vi "4Pi Objective Lock - EMBL.vi"(7 "Calling VI Ref":refnum<vi>) -> ()   [LabVIEW 2016]
uses:
  <vilib>/Utility/miscctls.llb/LVPointTypeDef.ctl
  4Pi Objective Lock Type Defs/4Pi Obj Lock - Notifier Type.ctl
  4Pi Objective Lock Type Defs/4Pi Obj Lock - Actions.ctl
  <vilib>/vision/Image Controls.llb/IMAQ Image.ctl
  4Pi Objective Lock Type Defs/4Pi Obj Lock - Lock Settings.ctl
  Hardware Configuration/Hardware Configuration Controls/Device Type.ctl
  Hardware Configuration/Hardware Configuration Controls/Device Function.ctl
  4Pi Objective Lock Type Defs/4Pi Obj Lock - Camera Settings.ctl
  Device Library/Cameras/Camera Controls/Generic Camera ROI.ctl
  Device Library/Cameras/Camera Controls/Generic Camera Actions.ctl
  Device Library/Stages/Stages Controls/Stage Actions.ctl
  <vilib>/addons/control/pid/pid.llb/PID (DBL Array).vi
  <vilib>/addons/control/pid/pid.llb/PID (DBL).vi
  <vilib>/addons/control/pid/NI_PID_pid.lvlib
  <vilib>/vision/NI_Vision_Development_Module.lvlib
panel:
  out "dt z (s)":dbl format="%.3f"
  out "dz (µm)":dbl format="%.2f"
  out "dxy (px)":dbl[](array[numeric])
  in  "Main Tab":T1(tab)
  out "Z Move":bool
  out "XY Move":bool
  out "Measured X Position (px)":dbl=1.0 format="%.3g"
  out "Measured Y Position (px)":dbl=1.0 format="%.3g"
  out "Measured sx/sy":dbl=1.0 format="%.3g"
  out "Target X Position (px)":dbl=1.0 format="%.3g"
  out "Target Y Position (px)":dbl=1.0 format="%.3g"
  out "Target sx/sy":dbl=1.0 format="%.3g"
  out "Z Axis Position (µm)":dbl=1.0 format="%.4g"
  out "Y Axis Position (µm)":dbl=1.0 format="%.2g"
  out "X Axis Position (µm)":dbl=1.0 format="%.2g"
  out "Z Target and Fit Value (µm)":T2(graph)
  in  "Start Lock":bool
  out "Y Target and Fit Position (µm)":T2(graph)
  out "X Target and Fit Position (µm)":T2(graph)
  in  "Restart Lock":bool
  out "Fit Error":bool
  out "Move Limit Error":bool
  out "Target Z (µm)":dbl=1.0 format="%.3g"
  out "Measured Z (µm)":dbl=1.0 format="%.3g"
  out "Target X Position cc (px)":dbl=1.0 format="%.3g"
  out "Measured X Position cc (px)":dbl=1.0 format="%.3g"
  out "Measured Y Position cc (px)":dbl=1.0 format="%.3g"
  out "Target Y Position cc (px)":dbl=1.0 format="%.3g"
  in  "pixel size (µm)":dbl=0.05
  in  "X Update Scale Factor":dbl=0.01
  in  "Y Update Scale Factor":dbl=0.01
  in  "Z Update Scale Factor":dbl=0.2
  in  "Sample Z Step No.":u32=2
  in  "Sample Z Step Size (µm)":dbl=2.0
  in  "Update Delay (ms)":i32=10
  in  "D (Derivative)":dbl
  in  "I (Integral)":dbl
  in  "P (Proportional)":dbl=2.0
  in  "Invert Z Axis":bool
  in  "XY Drift Threshold":dbl=0.05
  in  "Abort If Error":bool
  in  "Flip XY Axis":bool
  in  "Invert X Axis":bool=TRUE
  in  "Invert Y Axis":bool=TRUE
  in  "Z Stage Move Limit (µm)":dbl=5.0
  in  "Z Drift Threshold":dbl=0.05
  in  "XY Stage Move Limit (µm)":dbl=1.0
  in  "Frame Accumulations":u16=10
  in  "XY Correction Active":bool=TRUE
  in  "Z Correction Active":bool=TRUE
  in  "Set Camera ROI":bool
  in  "Save Lock Settings":bool
  in  "Quit":bool
  # "Z Drift Settings"
  # "Camera Setup"
  # "XY Drift Settings"
  # "PID Control Values"
  # "General Settings"
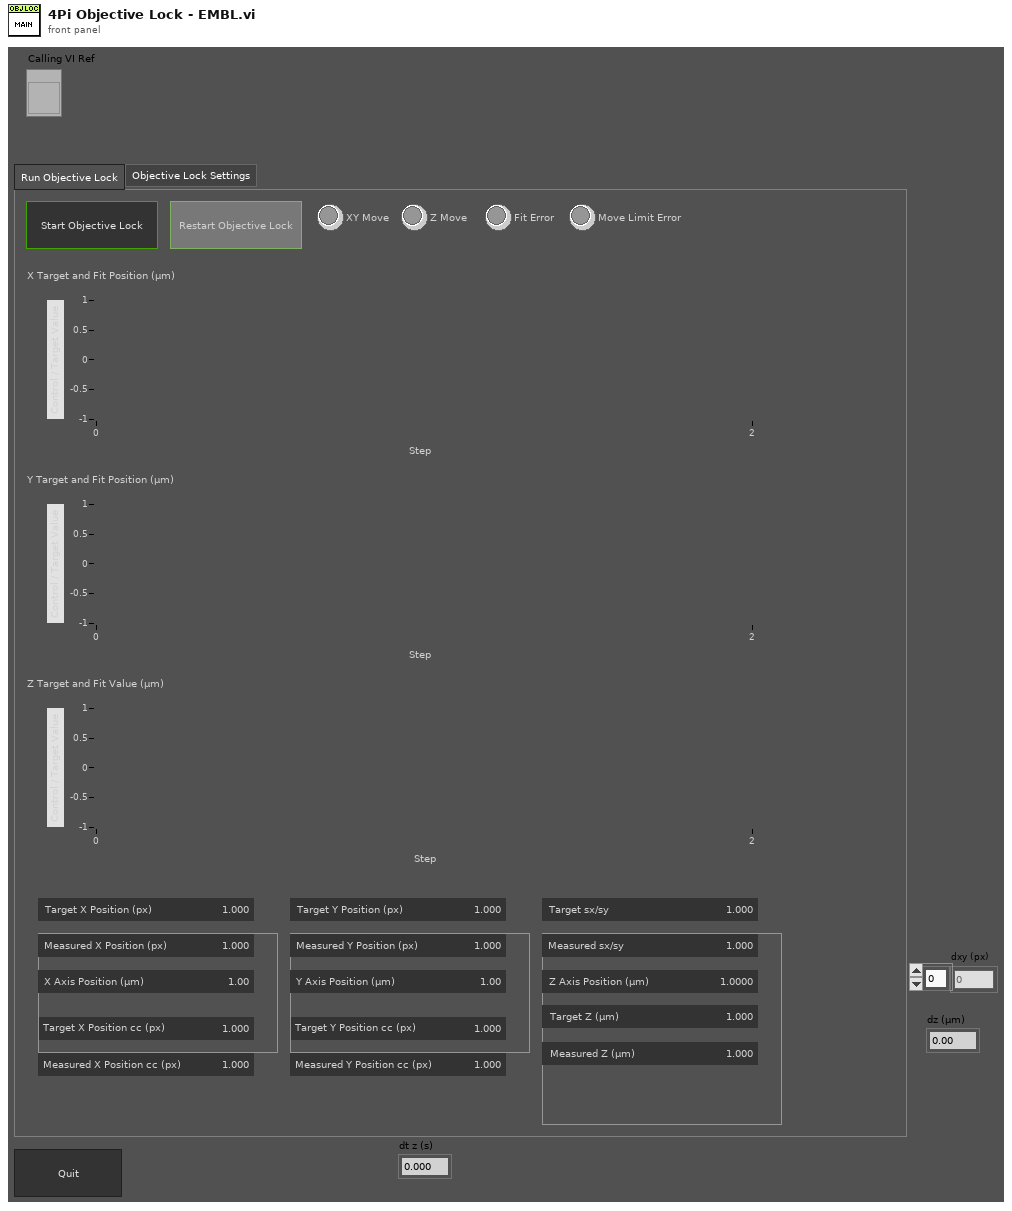
[diagram p1: front panel]
types:
  T1 = enum32{"Run Objective Lock", "Objective Lock Settings"}
  T2 = cluster{"Target 01":dbl, dbl, dbl, "Current 01":dbl, "Stage Pos":dbl, "Current 2":dbl}
  T3 = typedef "4Pi Obj Lock - Camera Settings.ctl" = cluster{"Exposure Time (s)":dbl, "H Offset":u16, "V Offset":u16, "H Width":u16, "V Width":u16}
  T4 = typedef "Device Function.ctl" = enum16{"Primary", "Secondary", "Overview", "Wide Field Drift Correction", "642 nm Excitation", "560 nm Excitation", "940 nm Excitation", "546 nm Excitation", "488 nm Excitation", "405 nm Excitation", "Objective Drift Correction", "4Pi Focus Lock", "4Pi Objective Lock", "Objective XY", "Objective Z", "Sample XY", "Sample Coarse Z", "Sample Z", "4Pi Lower", "4Pi Upper", "Em Small", "Em Large", "Ex Small", "Ex Large", "Mojo", "Adj Cavity", "Line Scanning", "Alert"}
  T5 = typedef "Device Type.ctl" = enum16{"AOTF", "Camera", "Deformable Mirror", "Laser", "Flip Mirror", "Shutter", "Stage", "Waveform", "FPGA", "Email"}
  T6 = typedef "4Pi Obj Lock - Actions.ctl" = enum16{"Idle", "Start Lock", "Restart Lock", "Get Initial Position", "Get Target Z Position", "Get Ref Stack", "Cal Ref FFT", "Move To Init Z", "Get Current Image", "Get Current Z Position", "Get Current XY Position", "Get Current Position", "Check Drift", "Check Drift cc xy", "Check Drift cc z", "Check Drift cc", "Move XYZ", "Move XY", "Move Z", "Update Plots", "Delay", "Abort", "Exit Loop", "Quit"}
  T7 = typedef "4Pi Obj Lock - Lock Settings.ctl" = cluster{"Z Drift Threshold":dbl, "Z Stage Move Limit (µm)":dbl, "XY Drift Threshold":dbl, "XY Stage Move Limit (µm)":dbl, "Frame Accumulations":u16, "Abort If Error":bool, "Flip XY Axis":bool, "Invert X Axis":bool, "Invert Y Axis":bool, "Invert Z Axis":bool, "Z Correction Active":bool, "XY Correction Active":bool, "PID Values":dbl[], "Update Delay (ms)":i32, "Sample Z Step Size (µm)":dbl, "Sample Z Step No.":u32, "Z Update Scale Factor":dbl, "Y Update Scale Factor":dbl, "X Update Scale Factor":dbl}
  T8 = typedef "4Pi Obj Lock - Notifier Type.ctl" = cluster{"Actions":T6, "Z Drift Threshold":dbl, "Z Stage Move Limit (µm)":dbl, "XY Drift Threshold":dbl, "XY Stage Move Limit (µm)":dbl, "Frame Accumulations":u16, "Abort If Error":bool, "Z Correction Active":bool, "XY Correction Active":bool, "PID Values":dbl[], "Running?":bool, "Update Delay (ms)":i32, "Cur Image (SGL)":T9, "Ref Stack (SGL)":T9[], "Sample Z (µm)":dbl[], "Initial Z Position (µm)":dbl, "Z Step Size (µm)":dbl, "Z Step No.":u32, "Ref FFT Stack (CSG)":T9[], "CC Image (SGL) ":T9, "Tmp Image FFT (CSG)":T9[], "CC Image Max (SGL)":T9}
  T9 = typedef "IMAQ Image.ctl" = refnum<image>
  T10 = enum16{"Always On", "Always Off", "Off While Running"}
  T11 = typedef "LVPointTypeDef.ctl" = cluster{"Horizontal":i16, "Vertical":i16}
  T12 = typedef "Image Type" = u32
  T13 = typedef "Generic Camera Actions.ctl" = enum16{"Status", "Live Preview", "Capture", "Abort", "Set Exposure Time (s)", "Get Exposure Time (s)", "Record Settings", "Set ROI", "Get ROI", "Defect Correction On/Off", "Cooler On/Off", "Fan On/Off", "Quit"}
  T14 = typedef "Generic Camera ROI.ctl" = cluster{"H_Offset":u16, "V_Offset":u16, "H_Width":u16, "V_Width":u16}
  T15 = typedef "Stage Actions.ctl" = enum16{"Get Position", "MVR", "MOVE", "HALT", "ONTARGET", "ERROR", "REFERENCE", "INIT", "VELOCITY", "STATUS", "EXIT", "HOME", "ZEROPOS", "NANOPOS", "ANALOG", "QUIT"}
  T16 = enum32{"Invalid", "Standard", "Closed", "Hidden", "Minimized", "Maximized"}
  T17 = cluster{"Target 01":dbl, dbl, dbl, "Current 01":dbl, "Stage Pos":dbl, "Current 2":dbl}[]
  T18 = typedef "Stage Status.ctl" = enum16{"Error", "Abort", "Busy", "On Target"}
  T19 = typedef "2D Gaussian - Best Fit Parameters.ctl" = cluster{"Amplitude":dbl, "X Position":dbl, "Y Position":dbl, "X Width":dbl, "Y Width":dbl, "Offset":dbl}
  T20 = cluster{"PID Values[0]":dbl, "PID Values[1]":dbl, "PID Values[2]":dbl}
  T21 = cluster{"PID Values[0]":dbl, "PID Values[1]":dbl, "PID Values[2]":dbl}[]
  T22 = typedef "LVRectTypeDef.ctl" = cluster{"Left":i16, "Top":i16, "Right":i16, "Bottom":i16}
  T23 = typedef "LVBoundsTypeDef.ctl" = cluster{"Width":u32, "Height":u32}
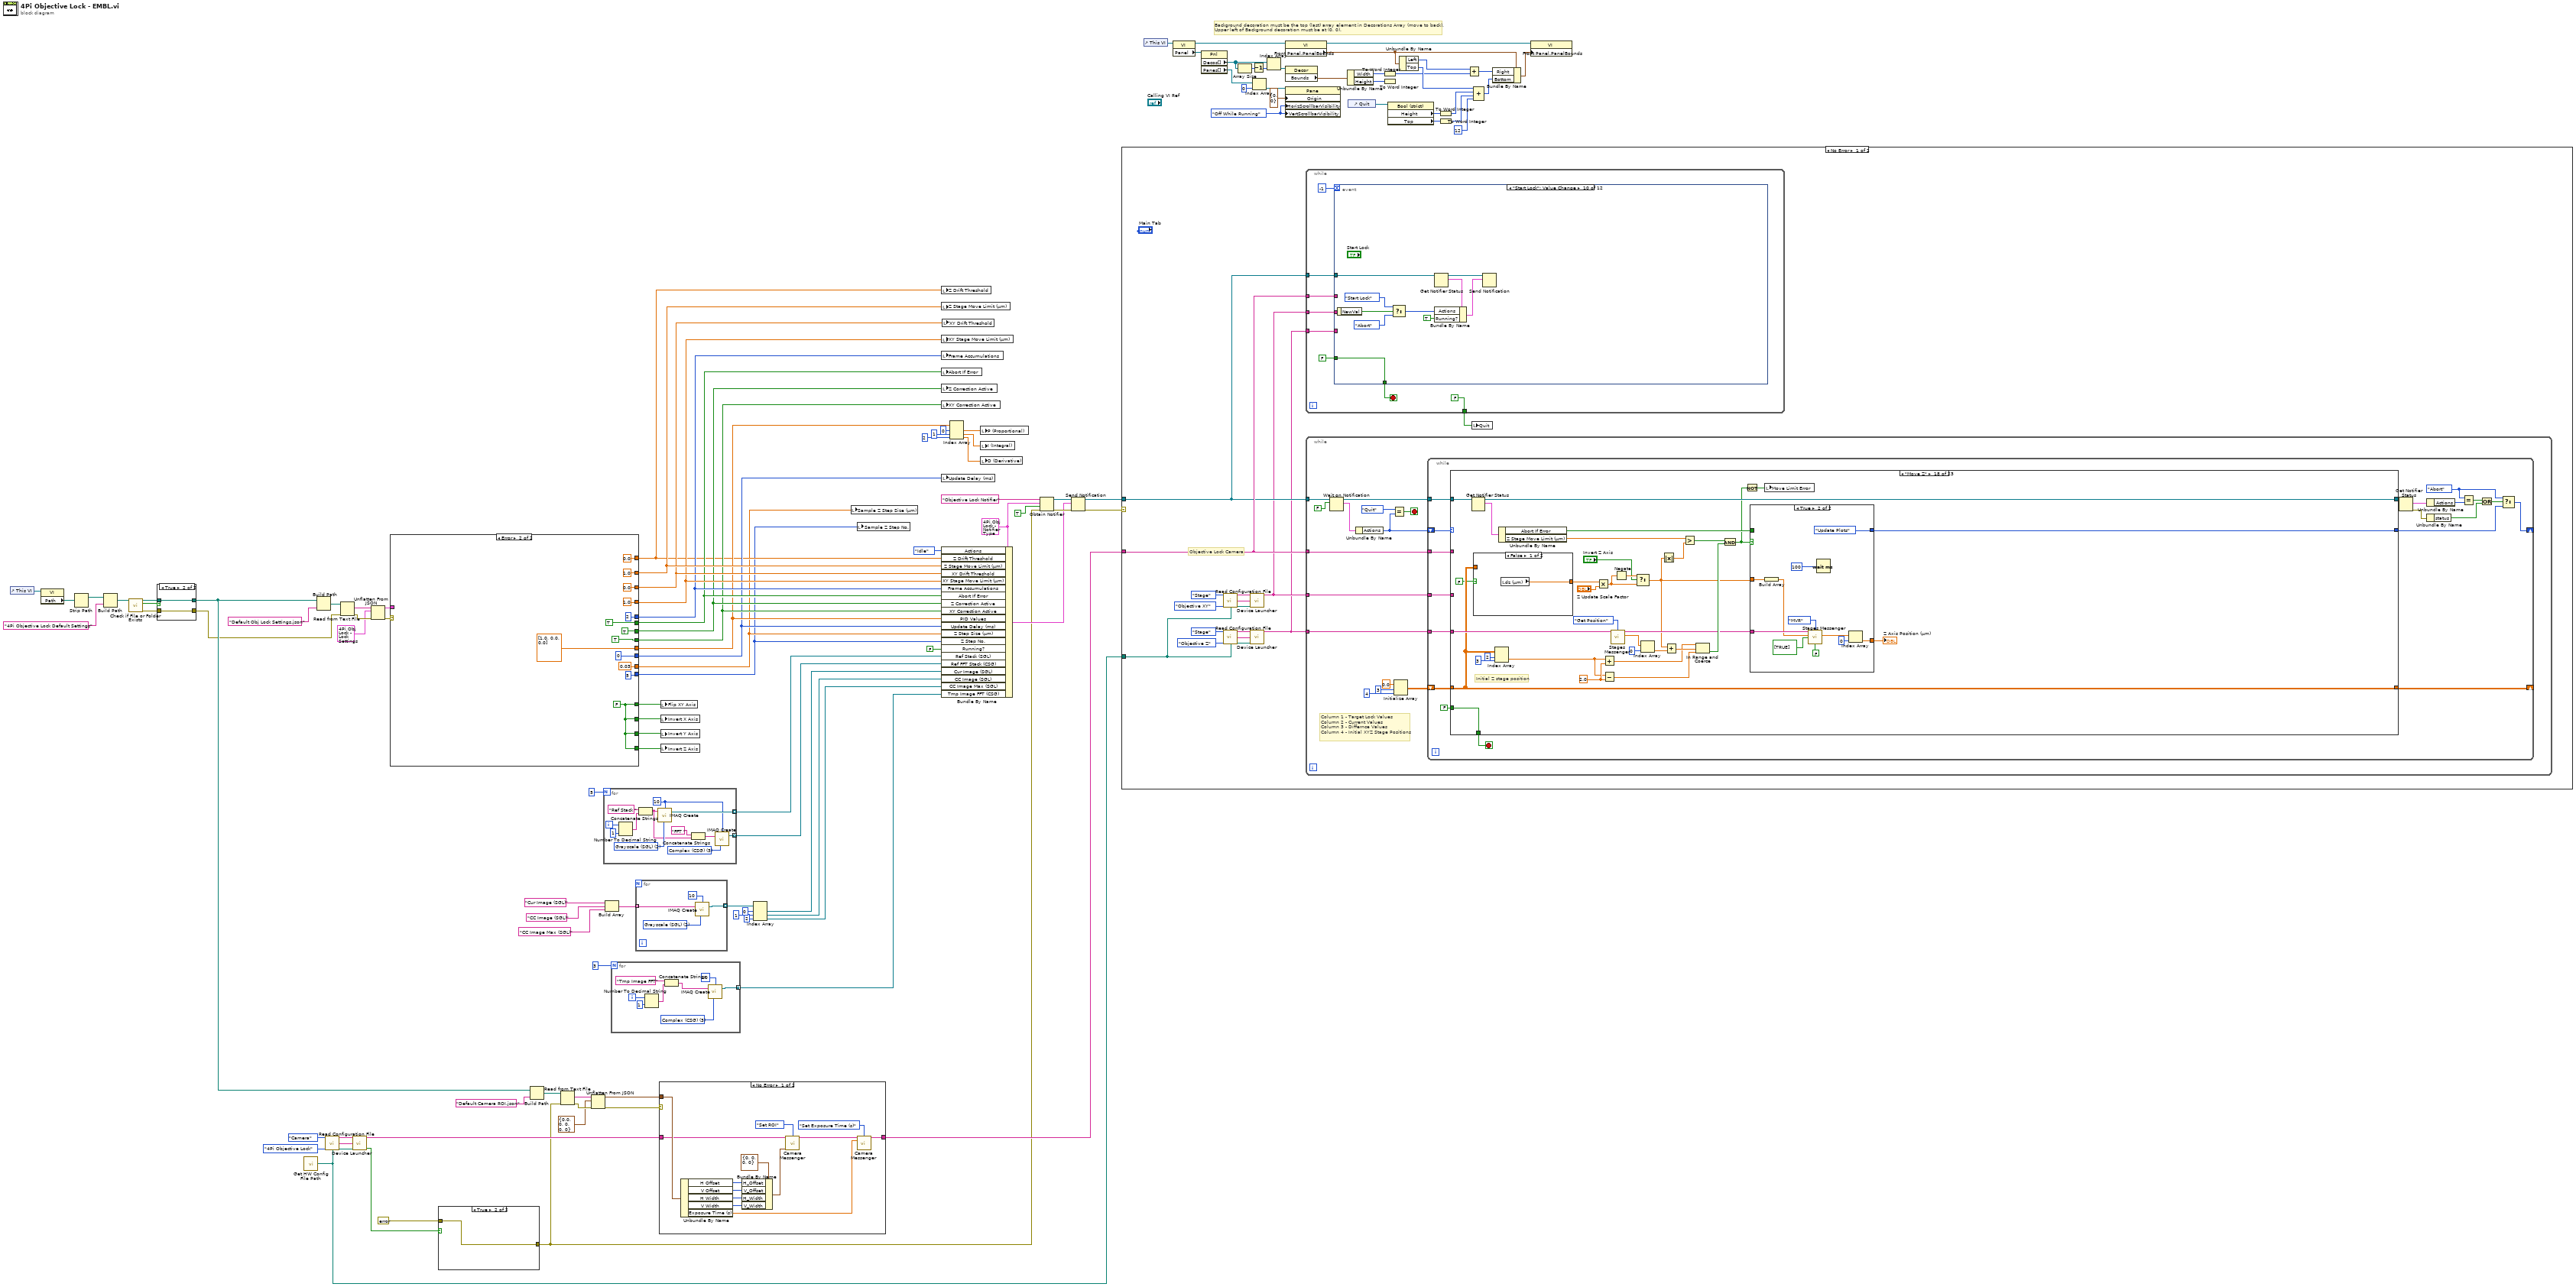
[diagram p0: block diagram]
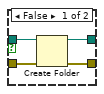
[diagram p2: hidden frame]
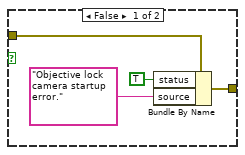
[diagram p3: hidden frame]
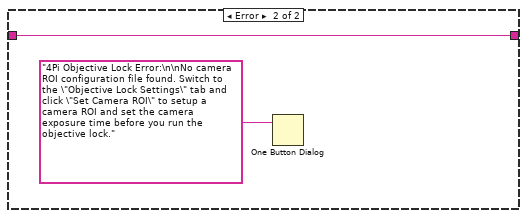
[diagram p4: hidden frame]
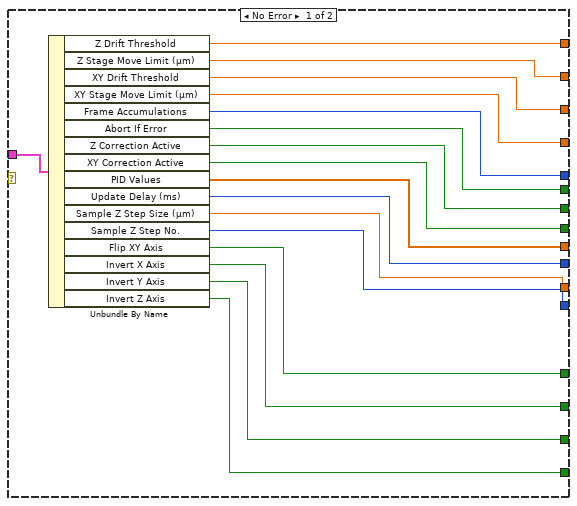
[diagram p5: hidden frame]
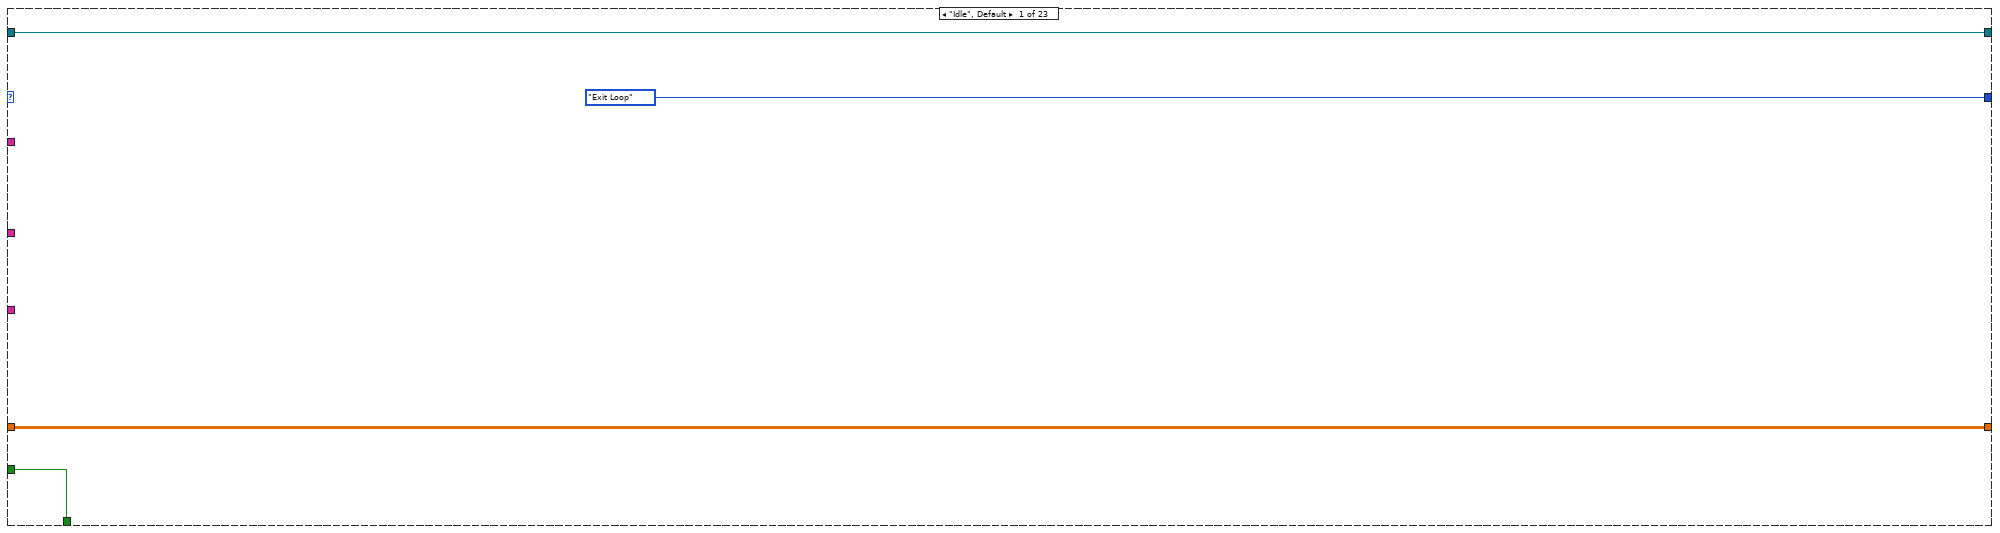
[diagram p6: hidden frame]
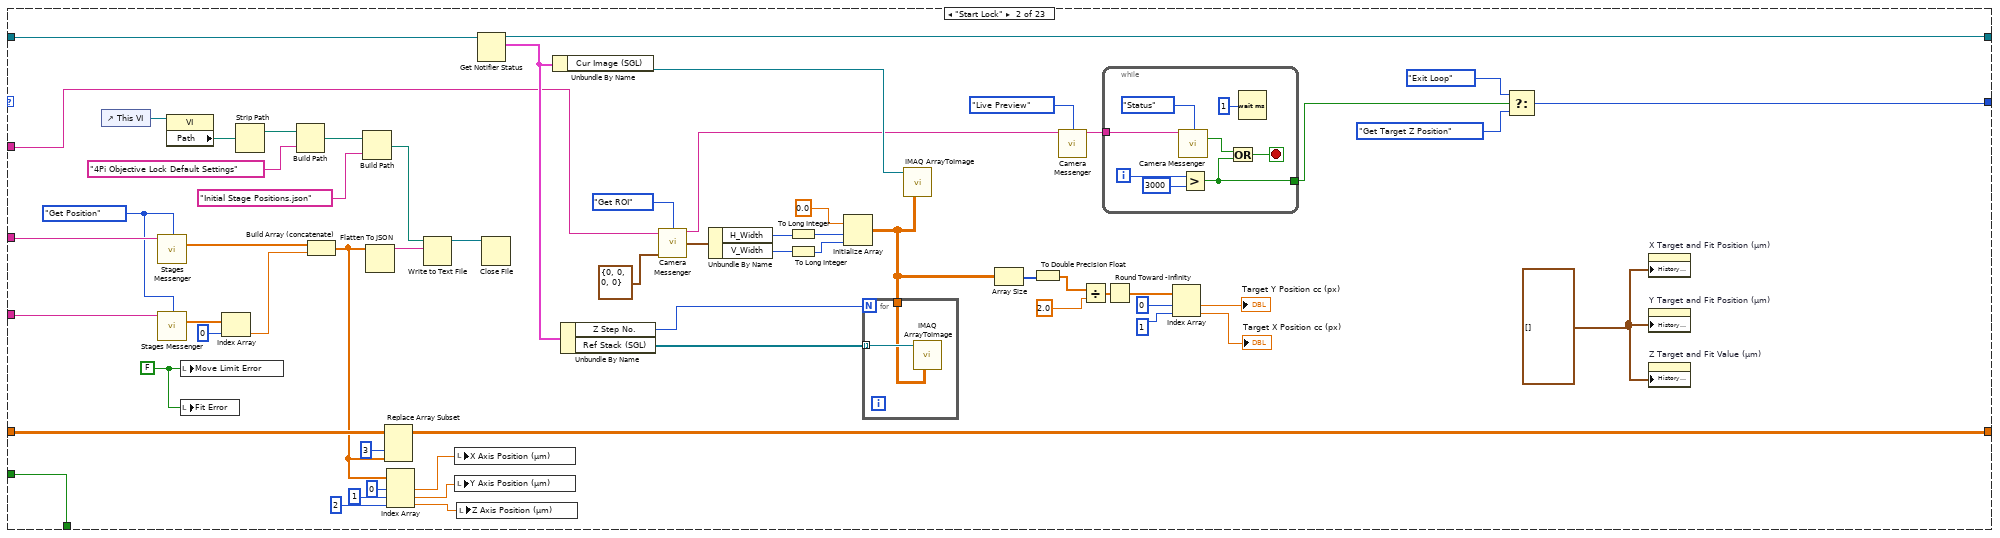
[diagram p7: hidden frame]
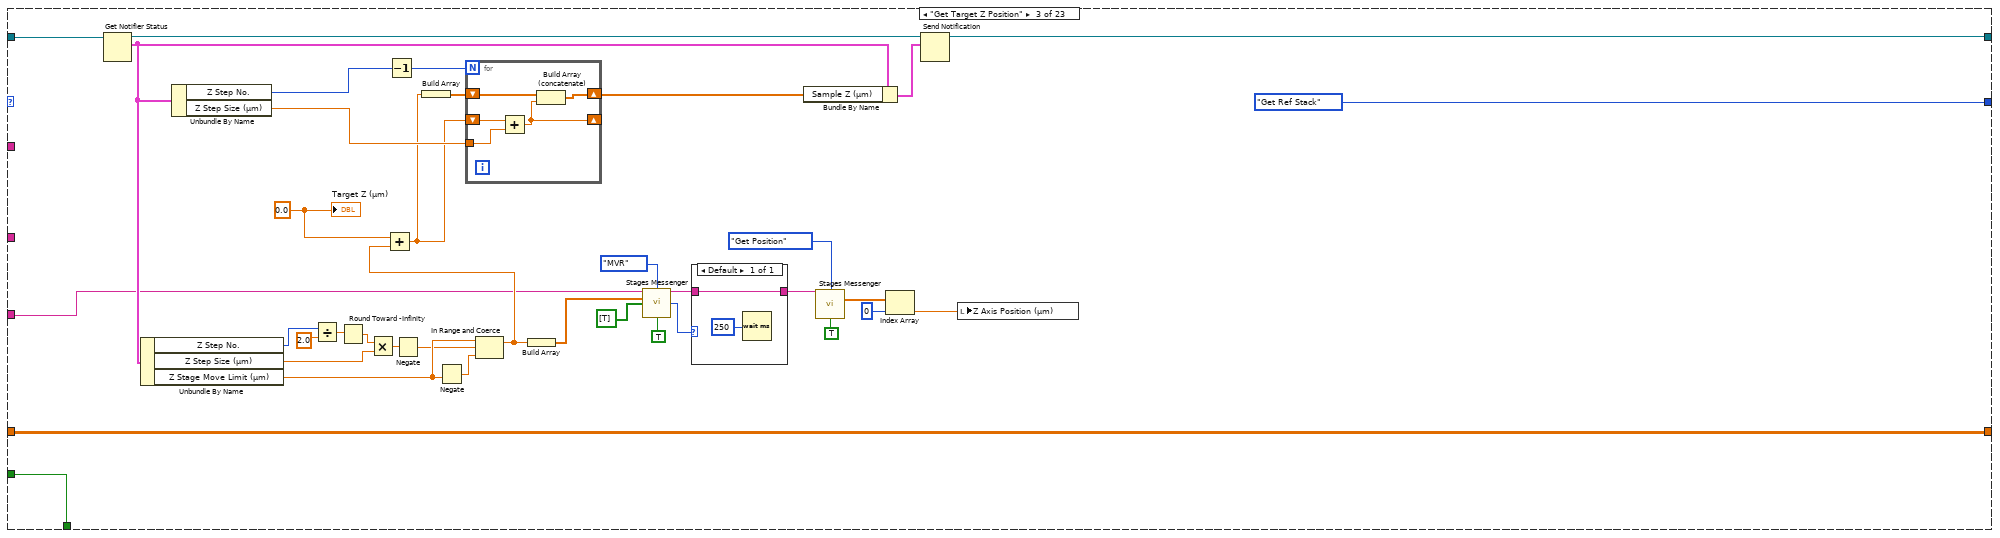
[diagram p8: hidden frame]
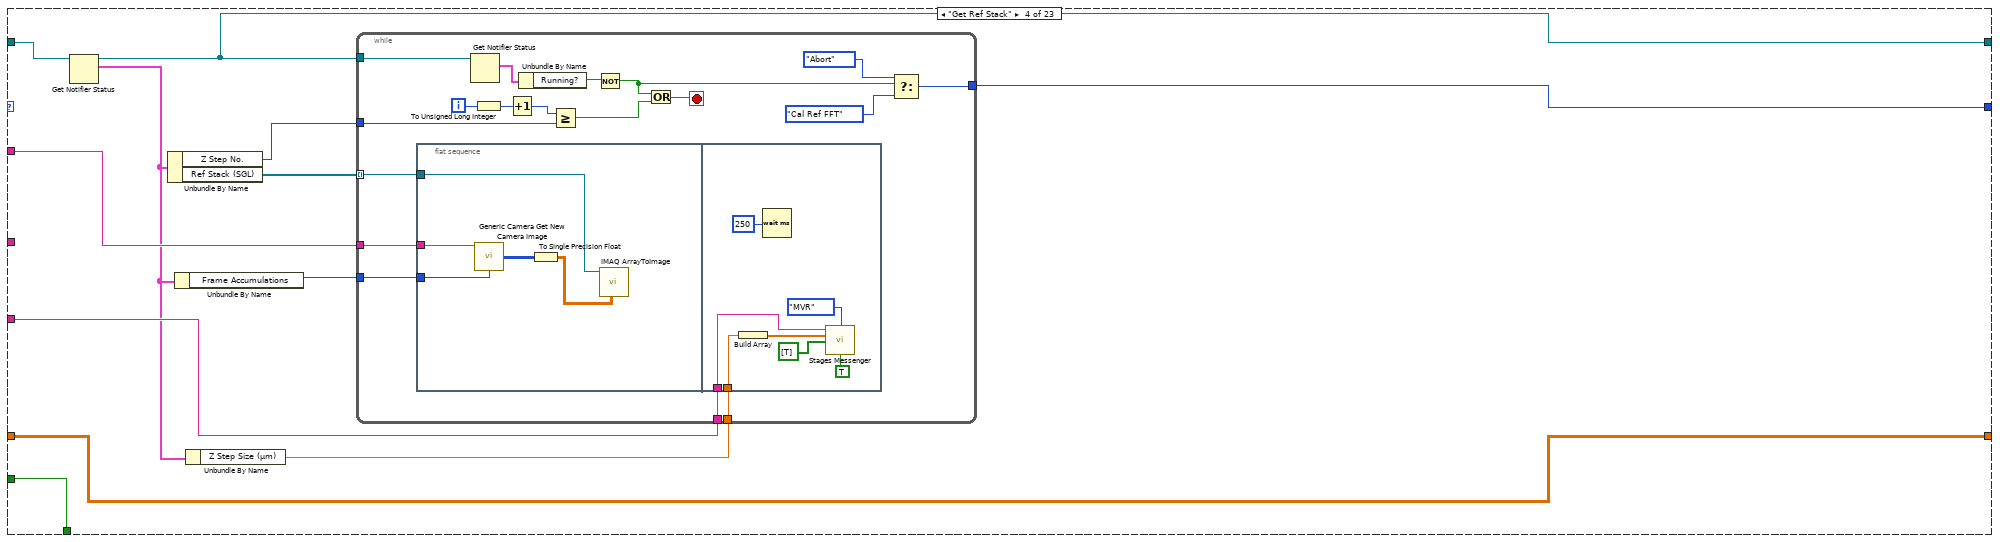
[diagram p9: hidden frame]
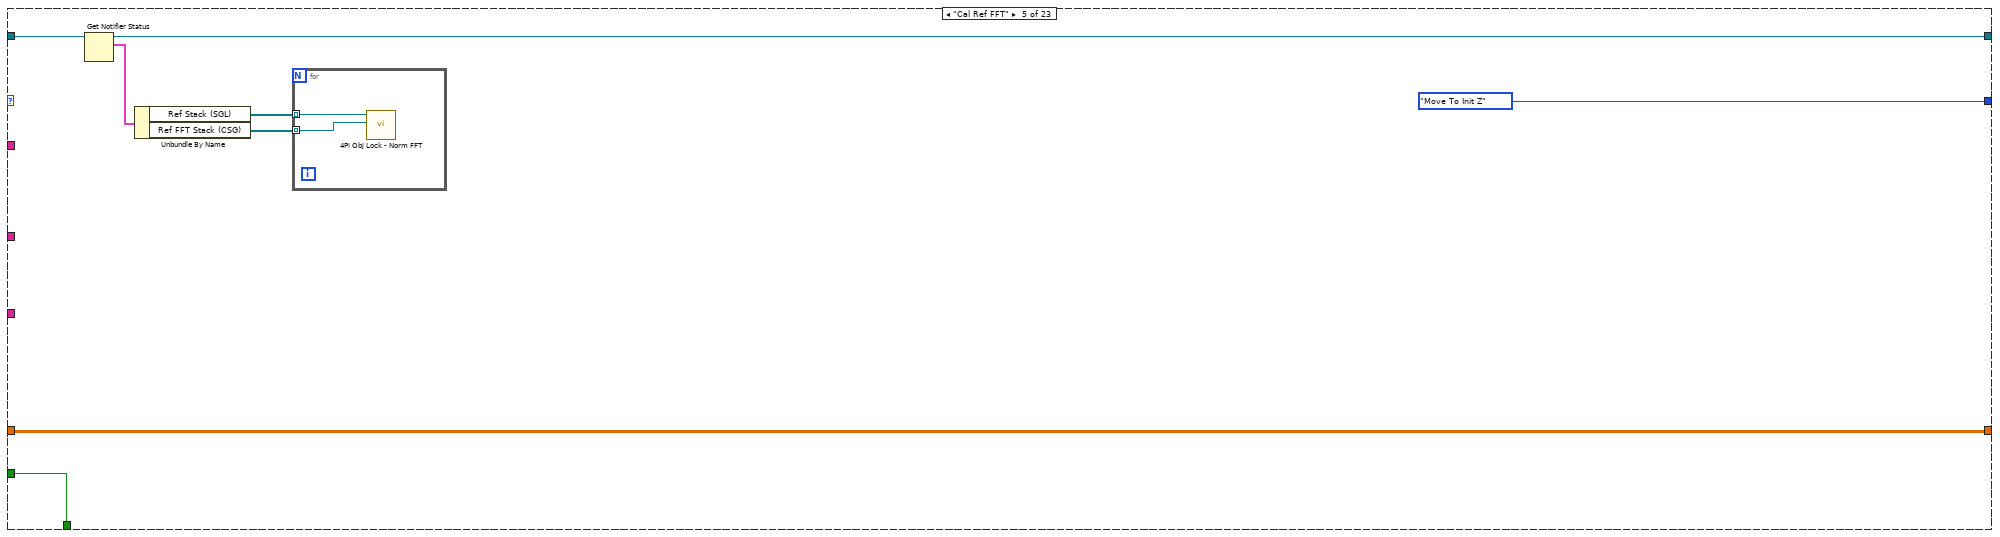
[diagram p10: hidden frame]
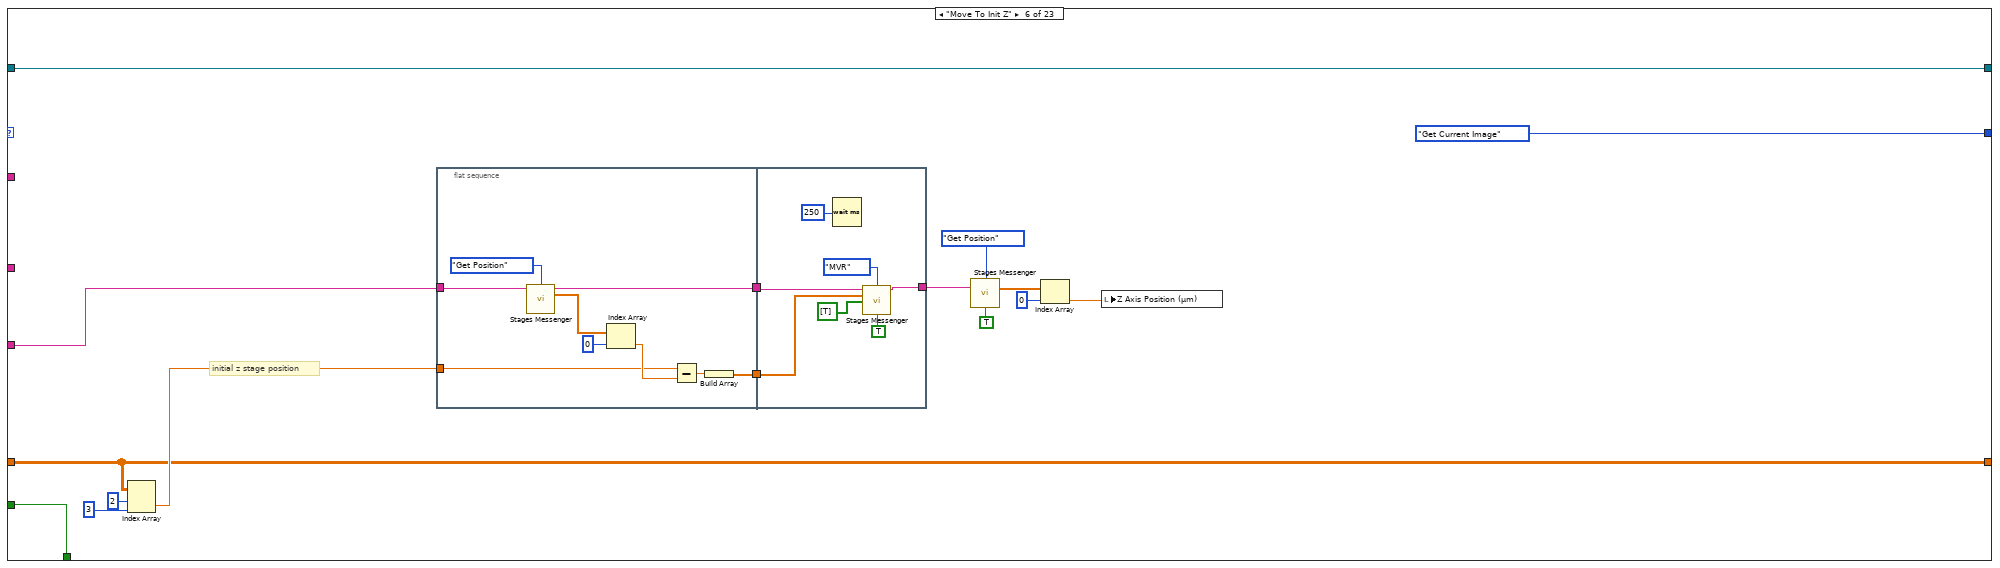
[diagram p11: hidden frame]
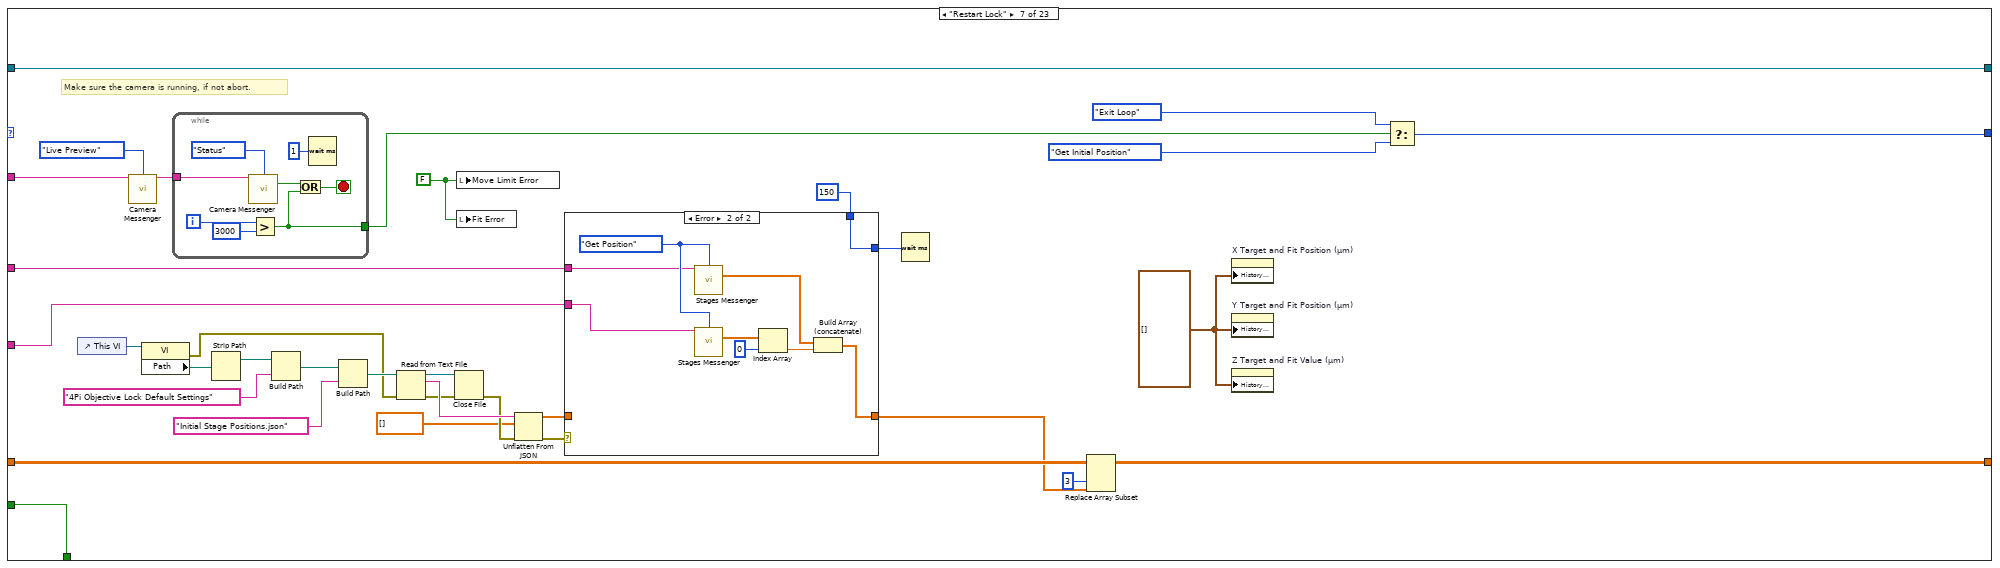
[diagram p12: hidden frame]
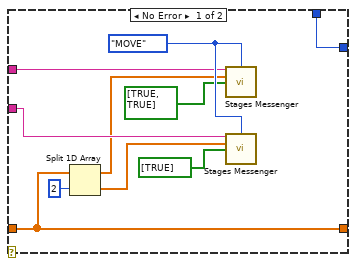
[diagram p13: hidden frame]
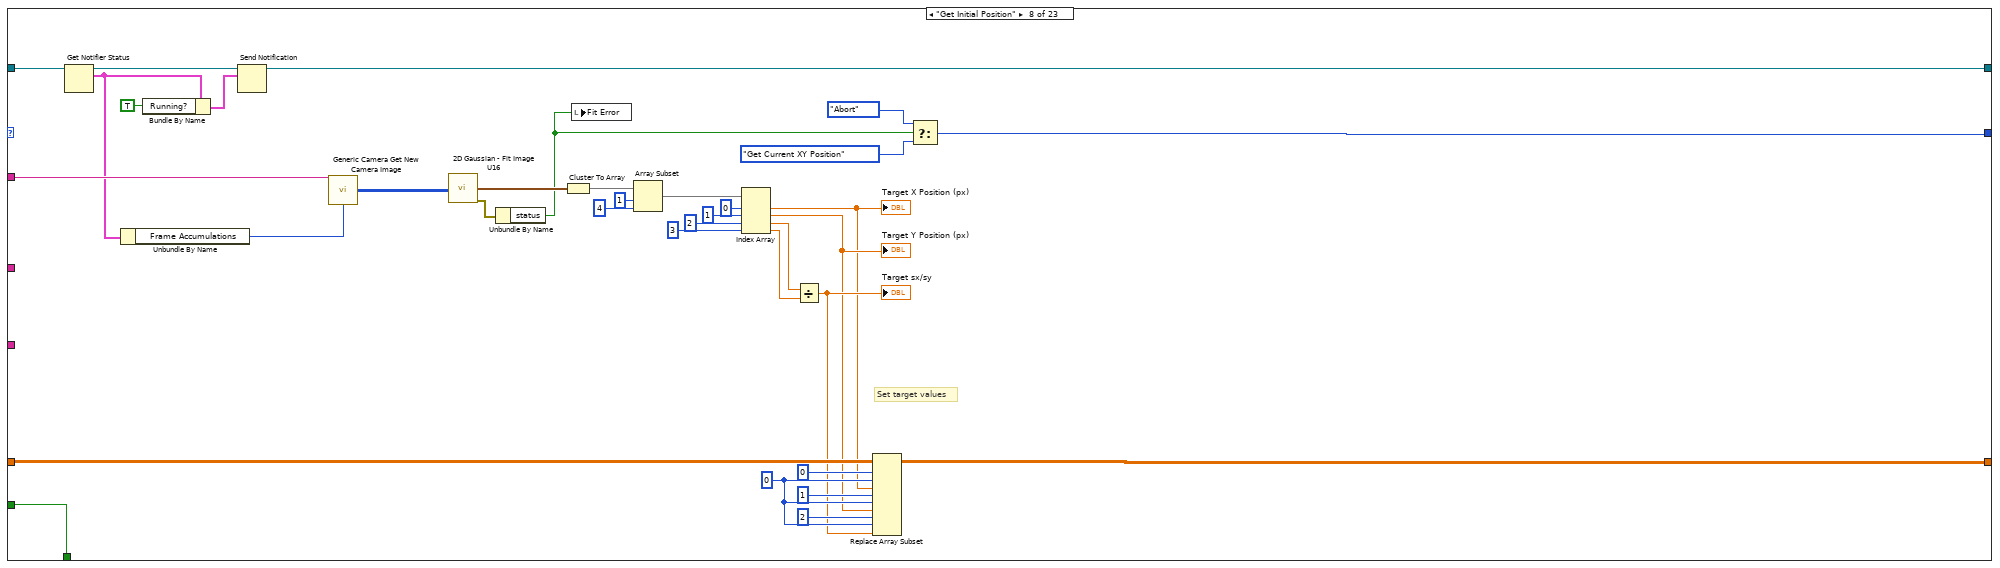
[diagram p14: hidden frame]
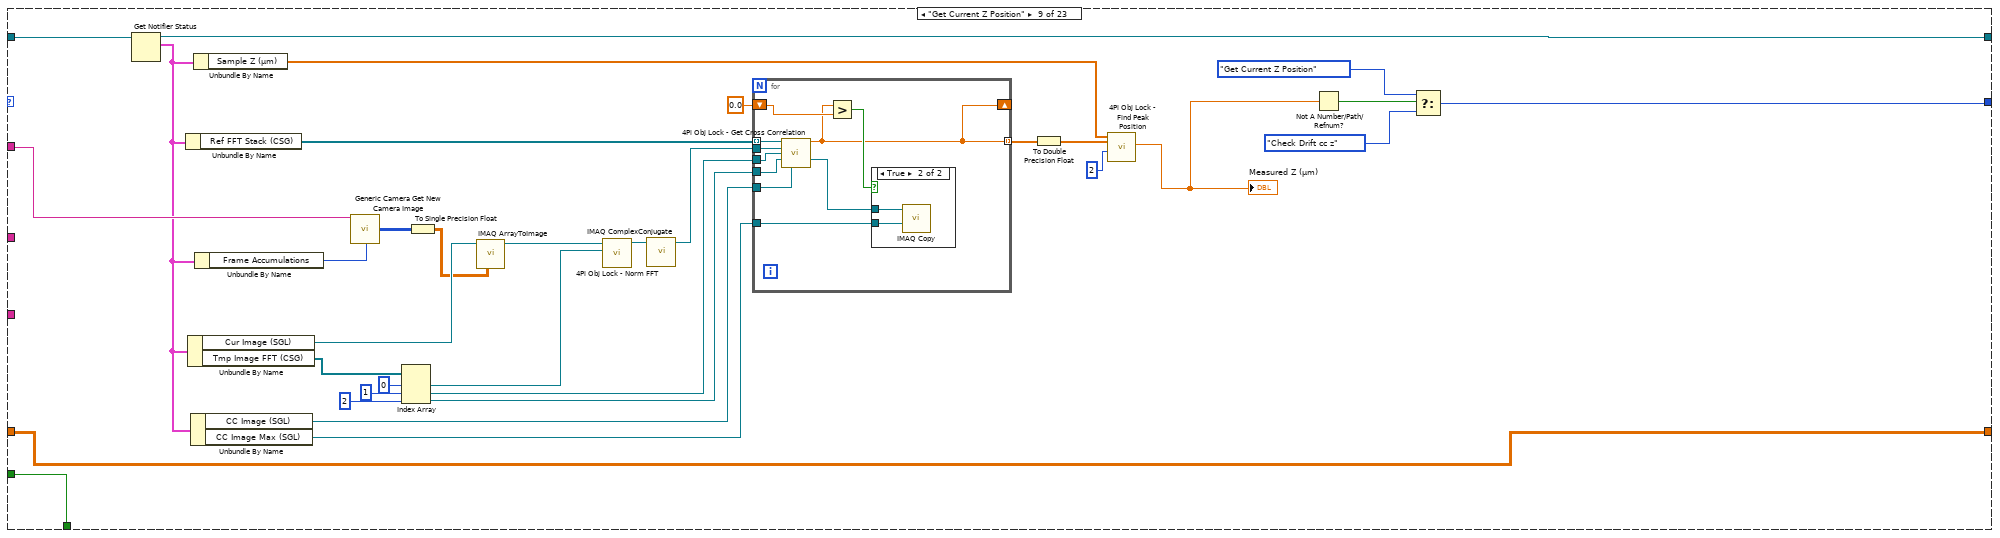
[diagram p15: hidden frame]
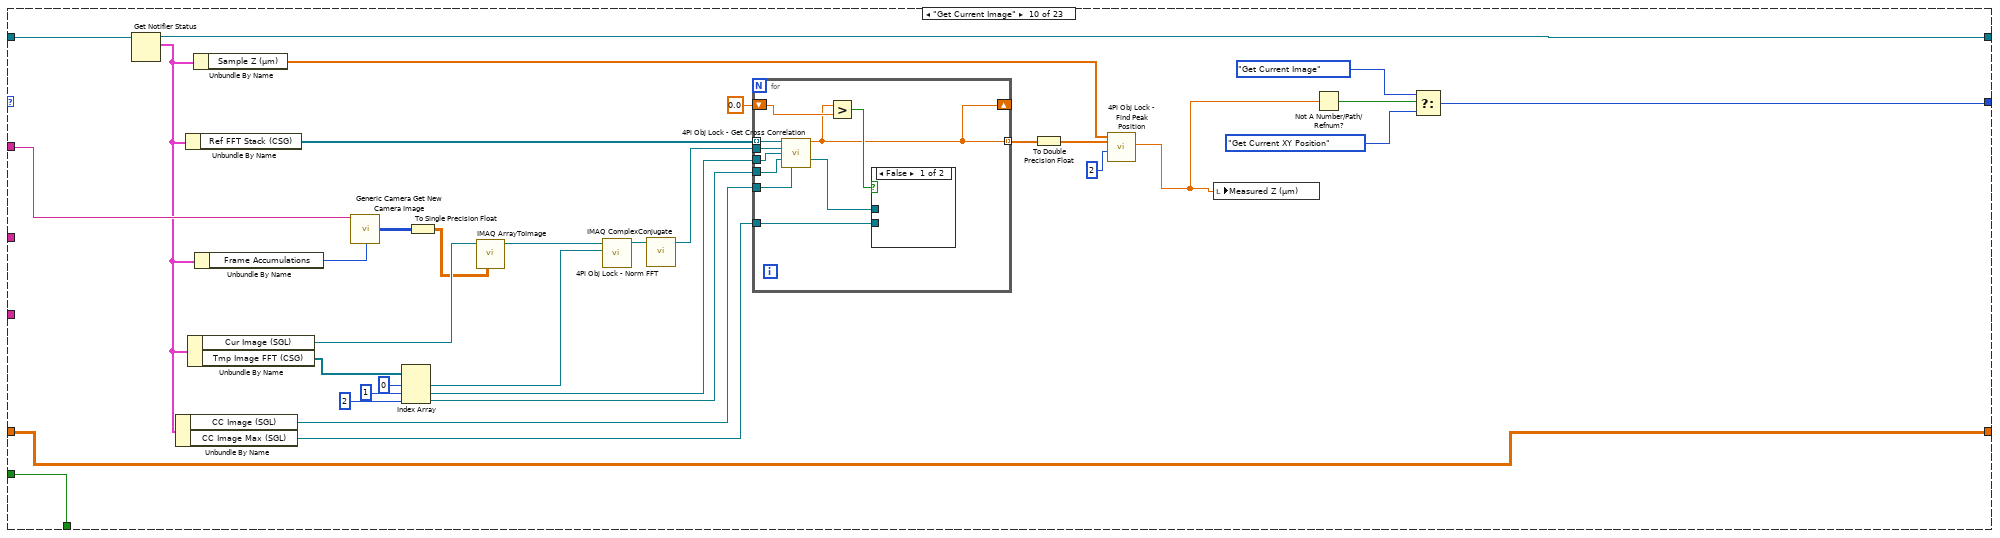
[diagram p17: hidden frame]
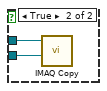
[diagram p18: hidden frame]
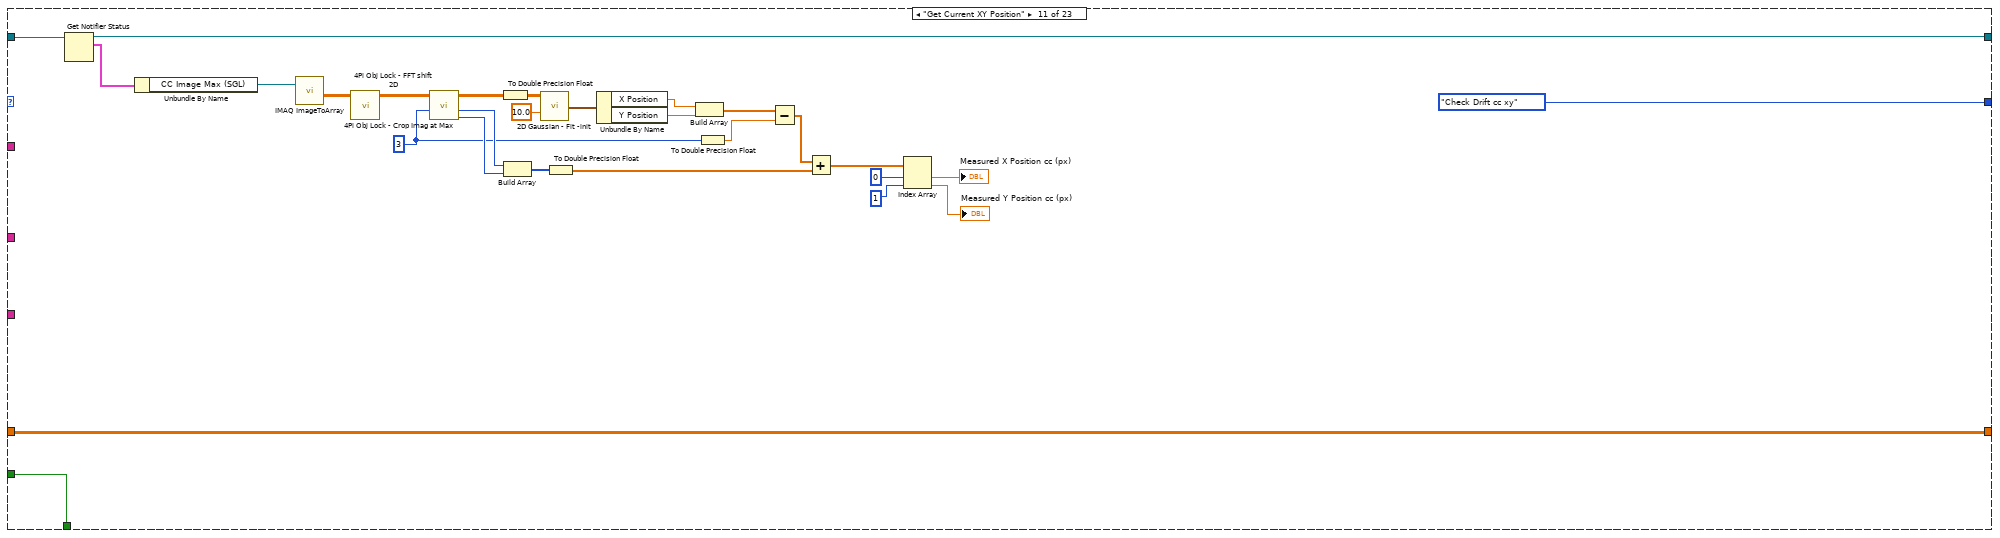
[diagram p19: hidden frame]
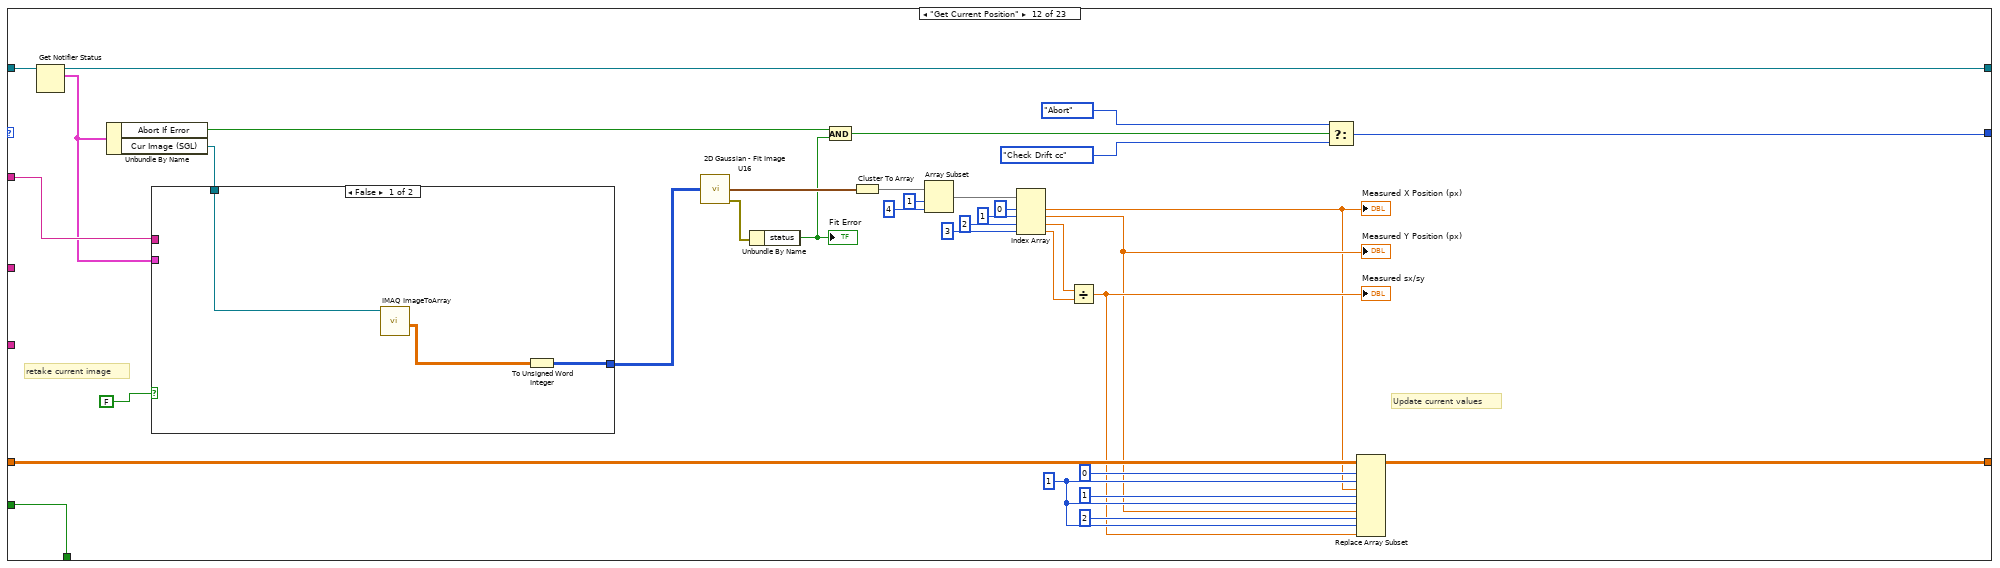
[diagram p20: hidden frame]
diagram:
  w78 = T8 {"Actions"=enum."Idle", "Z Drift Threshold"=0.05, "Z Stage Move Limit (µm)"=1.0, "XY Drift Threshold"=0.05, "XY Stage Move Limit (µm)"=1.0, "Frame Accumulations"=10, "Abort If Error"=FALSE, "Z Correction Active"=FALSE, "XY Correction Active"=FALSE, "PID Values"=[], "Running?"=FALSE, "Update Delay (ms)"=0, "Cur Image (SGL)"=refnum, "Ref Stack (SGL)"=[], "Sample Z (µm)"=[], "Initial Z Position (µm)"=0.0, "Z Step Size (µm)"=2.0, "Z Step No."=2, "Ref FFT Stack (CSG)"=[], "CC Image (SGL) "=refnum, "Tmp Image FFT (CSG)"=[], "CC Image Max (SGL)"=refnum} ("4Pi Obj Lock")
  w95 = T10."Off While Running" ("Vertical Scrollbar Visibility")
  # "Background decoration must be the top (last) array element in Decorations Array (move to back).\nUpper left of Background decoration must be at (0, 0)."
  n1 = control-ref of="This VI"() -> (w66:refnum<vi>)
  n2 = property class="VI"(reference=w66) -> ("Path"=w48:path)  [unwired: 1 in, 2 out]
  n3 = Strip Path(path=w48) -> (stripped path=w47:path)  [unwired: 1 out]
  n4 = Build Path(base path=w47, name or relative path="4Pi Objective Lock Default Settings") -> (appended path=w24:path)
  n5 = call <vilib>:"Check if File or Folder Exists.vi"("path"=w24) -> ("error out"=w20:errorcluster, "file or folder exists?"=w23:bool, "dup path"=w22:path)  [unwired: 8 in]
  n6 = case shown="True" w23 {
    tunnel: w22 -> [w116 w118]
    tunnel: [w115 w118] -> w21
    tunnel: w20 -> [w114 w117]
    tunnel: [w113 w117] -> w19
    frame False {
      n7 = Create Folder(path (use dialog)=w116, error in=w114) -> (created path=w115:path, error out=w113:errorcluster)  [unwired: 1 in, 1 out]
    }
    frame True {
    }
  }
  n8 = call "Get HW Config File Path.vi"() -> ("File Path"=w56:path)  [unwired: 14 in, 1 out]
  n9 = Build Path(base path=w21, name or relative path="Default Obj Lock Settings.json") -> (appended path=w75:path)
  n10 = call "Read Configuration File.vi"("Device Type"=Device_Type."Camera", "Device Function"=Device_Function."4Pi Objective Lock", "Config File Path"=w56) -> ("Unique Notifier Name"=w63:string, "Device Ports/IDs/Channels"=w65:string[], "Device Engine Path"=w64:path)  [unwired: 9 in, 1 out]
  n11 = Read from Text File(file (use dialog)=w75, error in=w19) -> (text=w74:string, error out=w73:errorcluster)  [unwired: 2 in, 2 out]
  n12 = call "Device Launcher.vi"("Notifier Name"=w63, "Device Ports/IDs/Channels"=w65, "Device Engine Path"=w64) -> ("Notifier Name"=w54:string, "Running?"=w60:bool)  [unwired: 11 in]
  n13 = Unflatten From JSON(JSON string=w74, type and defaults=T7 {"Z Drift Threshold"=0.05, "Z Stage Move Limit (µm)"=1.0, "XY Drift Threshold"=0.05, "XY Stage Move Limit (µm)"=1.0, "Frame Accumulations"=10, "Abort If Error"=FALSE, "Flip XY Axis"=FALSE, "Invert X Axis"=FALSE, "Invert Y Axis"=FALSE, "Invert Z Axis"=FALSE, "Z Correction Active"=TRUE, "XY Correction Active"=TRUE, "PID Values"=[], "Update Delay (ms)"=0, "Sample Z Step Size (µm)"=2.0, "Sample Z Step No."=2, "Z Update Scale Factor"=2.0, "Y Update Scale Factor"=2.0, "X Update Scale Factor"=2.0} ("Lock Settings"), error in (no error)=w73) -> (value=w70:T7, error out=w71:errorcluster)  [unwired: 4 in]
  n14 = case shown="Error" w71 {
    tunnel: [w134 0.0 ("Z Drift Threshold")] -> w25
    tunnel: [w133 1.0 ("Z Stage Move Limit (µm)")] -> w40
    tunnel: [w131 0.0 ("XY Drift Threshold")] -> w39
    tunnel: [w132 1.0 ("XY Stage Move Limit (µm)")] -> w38
    tunnel: [w130 u16 2 ("Frame Accumulations")] -> w37
    tunnel: [w129 TRUE ("Abort If Error")] -> w36
    tunnel: w70 -> [w135 _]
    tunnel: [w128 TRUE ("Z Correction Active")] -> w35
    tunnel: [w127 TRUE ("XY Correction Active")] -> w34
    tunnel: [w126 dbl[] [1.0, 0.0, 0.0] ("PID Values")] -> w33
    tunnel: [w125 u16 0 ("Update Delay (ms)")] -> w26
    tunnel: [w124 w138] -> w42
    tunnel: [w123 w138] -> w43
    tunnel: [w122 w138] -> w44
    tunnel: [w121 w138] -> w45
    tunnel: [w120 0.03 ("Sample Z Step Size (µm)")] -> w5
    tunnel: [w119 u32 5 ("Sample Z Step No.")] -> w4
    frame No Error {
      n15 = Unbundle By Name(w135) -> ("Z Drift Threshold"=w134:dbl, "Z Stage Move Limit (µm)"=w133:dbl, "XY Drift Threshold"=w131:dbl, "XY Stage Move Limit (µm)"=w132:dbl, "Frame Accumulations"=w130:u16, "Abort If Error"=w129:bool, "Z Correction Active"=w128:bool, "XY Correction Active"=w127:bool, "PID Values"=w126:dbl[], "Update Delay (ms)"=w125:i32, "Sample Z Step Size (µm)"=w120:dbl, "Sample Z Step No."=w119:u32, "Flip XY Axis"=w121:bool, "Invert X Axis"=w122:bool, "Invert Y Axis"=w123:bool, "Invert Z Axis"=w124:bool)
    }
    frame Error {
      w138 = FALSE ("Flip XY Axis")
    }
  }
  n16 = case shown="True" w60 {
    tunnel: errorcluster {"status"=FALSE, "code"=0, "source"=""} ("Error") -> [w152 w153]
    tunnel: [w149 w153] -> w46
    frame False {
      n17 = Bundle By Name(cluster=w152, "status"=TRUE, "source"="Objective lock camera startup error." ("name or relative path")) -> (w149:errorcluster)
    }
    frame True {
    }
  }
  n18 = Build Path(base path=w21, name or relative path="Default Camera ROI.json") -> (appended path=w50:path)
  n19 = Read from Text File(file (use dialog)=w50, error in=w46) -> (text=w68:string, error out=w67:errorcluster)  [unwired: 2 in, 2 out]
  n20 = Unflatten From JSON(JSON string=w68, type and defaults=T3 {"Exposure Time (s)"=0.0, "H Offset"=0, "V Offset"=0, "H Width"=0, "V Width"=0} ("Camera Settings"), error in (no error)=w67) -> (value=w53:T3, error out=w58:errorcluster)  [unwired: 4 in]
  n21 = for {
    N: 5 -> [_]
    tunnel: [w165] -> w17 mode=indexing
    tunnel: [w154] -> w16 mode=indexing
    i -> [w164]
    w159 = T12 3 items=["Grayscale (U8)", "Grayscale (I16)", "Grayscale (SGL)", "Complex (CSG)", "RGB (U32)", "HSL (U32)", "RGB (U64)", "Grayscale (U16)"] ("Image Type")
    w160 = T12 2 items=["Grayscale (U8)", "Grayscale (I16)", "Grayscale (SGL)", "Complex (CSG)", "RGB (U32)", "HSL (U32)", "RGB (U64)", "Grayscale (U16)"] ("Image Type")
    w156 = 10 ("Border Size")
    n22 = Number To Decimal String(number=w164, width (-)=i16 1) -> (decimal integer string=w162:string)
    n23 = Concatenate Strings("Ref Stack " ("string"), w162) -> (w155:string)
    n24 = call "IMAQ Create"("Border Size"=w156, "Image Name"=w155, "Image Type"=w160) -> ("New Image"=w165:T9)  [unwired: 2 in, 1 out]
    n25 = Concatenate Strings("FFT " ("string"), w155) -> (w158:string)
    n26 = call "IMAQ Create"("Border Size"=w156, "Image Name"=w158, "Image Type"=w159) -> ("New Image"=w154:T9)  [unwired: 2 in, 1 out]
  }
  n27 = Build Array("Cur Image (SGL)" ("Image Name"), "CC Image (SGL)" ("Image Name"), "CC Image Max (SGL)" ("Image Name")) -> (w11:string[])
  n28 = for {
    N: 3 -> [_]
    tunnel: [w171] -> w6 mode=indexing
    i -> [w167]
    w172 = T12 3 items=["Grayscale (U8)", "Grayscale (I16)", "Grayscale (SGL)", "Complex (CSG)", "RGB (U32)", "HSL (U32)", "RGB (U64)", "Grayscale (U16)"] ("Image Type")
    n29 = Number To Decimal String(number=w167, width (-)=i16 1) -> (decimal integer string=w170:string)
    n30 = Concatenate Strings("Tmp Image FFT" ("Image Name"), w170) -> (w166:string)
    n31 = call "IMAQ Create"("Border Size"=10, "Image Name"=w166, "Image Type"=w172) -> ("New Image"=w171:T9)  [unwired: 2 in, 1 out]
  }
  n32 = for {
    tunnel: w11 -> [w175] mode=indexing
    tunnel: [w174] -> w10 mode=indexing
    w176 = T12 2 items=["Grayscale (U8)", "Grayscale (I16)", "Grayscale (SGL)", "Complex (CSG)", "RGB (U32)", "HSL (U32)", "RGB (U64)", "Grayscale (U16)"] ("Image Type")
    n33 = call "IMAQ Create"("Border Size"=10, "Image Name"=w175, "Image Type"=w176) -> ("New Image"=w174:T9)  [unwired: 2 in, 1 out]
  }
  n34 = case shown="No Error" w58 {
    tunnel: w54 -> [w181 w192]
    tunnel: w53 -> [w190 _]
    tunnel: [w178 w192] -> w52
    frame No Error {
      n35 = Unbundle By Name(w190) -> ("H Offset"=w185:u16, "V Offset"=w186:u16, "H Width"=w187:u16, "V Width"=w188:u16, "Exposure Time (s)"=w180:dbl)
      n36 = Bundle By Name(cluster=T14 {"H_Offset"=0, "V_Offset"=0, "H_Width"=0, "V_Width"=0} ("General Camera ROI"), "H_Offset"=w185, "V_Offset"=w186, "H_Width"=w187, "V_Width"=w188) -> (w184:T14)
      n37 = call "Camera Messenger.vi"("Notifier Name"=w181, "General Camera Actions"=Generic_Camera_Actions."Set ROI", "Camera ROI"=w184) -> ("Notifier Name Dup"=w179:string)  [unwired: 7 in, 5 out]
      n38 = call "Camera Messenger.vi"("Notifier Name"=w179, "General Camera Actions"=Generic_Camera_Actions."Set Exposure Time (s)", "Exposure Time (s)"=w180) -> ("Notifier Name Dup"=w178:string)  [unwired: 7 in, 5 out]
    }
    frame Error {
      n39 = One Button Dialog(message="4Pi Objective Lock Error:\n\nNo camera ROI configuration file found. Switch to the \"Objective Lock Settings\" tab and click \"Set Camera ROI\" to setup a camera ROI and set the camera exposure time before you run the objective lock.") -> ()  [unwired: 1 in, 1 out]
    }
  }
  n40 = local write "Flip XY Axis"(w45) -> ()
  n41 = local write "Invert X Axis"(w44) -> ()
  n42 = local write "Invert Y Axis"(w43) -> ()
  n43 = local write "Invert Z Axis"(w42) -> ()
  n44 = Index Array(array=w10, index #1=0 ("index"), index #2=1 ("index"), index #3=2 ("index")) -> (element #1=w9:T9, element #2=w8:T9, element #3=w1:T9)
  n45 = local write "Sample Z Step Size (µm)"(w5) -> ()
  n46 = local write "Sample Z Step No."(w4) -> ()
  n47 = Bundle By Name(cluster=w78, "Actions"=4Pi_Obj_Lock_-_Actions."Idle", "Z Drift Threshold"=w25, "Z Stage Move Limit (µm)"=w40, "XY Drift Threshold"=w39, "XY Stage Move Limit (µm)"=w38, "Frame Accumulations"=w37, "Abort If Error"=w36, "Z Correction Active"=w35, "XY Correction Active"=w34, "PID Values"=w33, "Update Delay (ms)"=w26, "Z Step Size (µm)"=w5, "Z Step No."=w4, "Running?"=FALSE ("Obj Lock Active?"), "Ref Stack (SGL)"=w17, "Ref FFT Stack (CSG)"=w16, "Cur Image (SGL)"=w9, "CC Image (SGL)"=w8, "CC Image Max (SGL)"=w1, "Tmp Image FFT (CSG)"=w6) -> (w77:T8)
  n48 = local write "Z Drift Threshold"(w25) -> ()
  n49 = local write "Z Stage Move Limit (µm)"(w40) -> ()
  n50 = local write "XY Stage Move Limit (µm)"(w38) -> ()
  n51 = local write "Frame Accumulations"(w37) -> ()
  n52 = local write "Abort If Error"(w36) -> ()
  n53 = local write "Z Correction Active"(w35) -> ()
  n54 = local write "XY Correction Active"(w34) -> ()
  n55 = local write "Update Delay (ms)"(w26) -> ()
  n56 = local write "XY Drift Threshold"(w39) -> ()
  n57 = Index Array(array=w33, index #1=0 ("index"), index #2=1 ("index"), index #3=2 ("index")) -> (element #1=w29:dbl, element #2=w27:dbl, element #3=w28:dbl)
  n58 = local write "P (Proportional)"(w29) -> ()
  n59 = local write "I (Integral)"(w27) -> ()
  n60 = local write "D (Derivative)"(w28) -> ()
  n61 = Obtain Notifier(name (unnamed)="Objective Lock Notifier", notification data type=w78, create if not found? (T)=TRUE, error in (no error)=w46) -> (notifier out=w80:refnum<notifier>, error out=w81:errorcluster)  [unwired: 1 out]
  n62 = Send Notification(notification=w77, notifier=w80, error in (no error)=w81) -> (notifier out=w79:refnum<notifier>, error out=w57:errorcluster)
  n63 = case shown="No Error" w57 {
    tunnel: w56 -> [w197 _]
    tunnel: w79 -> [w195 _]
    tunnel: w52 -> [w196 _]
    frame No Error {
      # "Objective Lock Camera"
      n64 = call "Read Configuration File.vi"("Device Type"=Device_Type."Stage", "Device Function"=Device_Function."Objective XY", "Config File Path"=w197) -> ("Unique Notifier Name"=w205:string, "Device Ports/IDs/Channels"=w203:string[], "Device Engine Path"=w204:path)  [unwired: 9 in, 1 out]
      n65 = call "Read Configuration File.vi"("Device Type"=Device_Type."Stage", "Device Function"=Device_Function."Objective Z", "Config File Path"=w197) -> ("Unique Notifier Name"=w200:string, "Device Ports/IDs/Channels"=w202:string[], "Device Engine Path"=w201:path)  [unwired: 9 in, 1 out]
      n66 = call "Device Launcher.vi"("Notifier Name"=w205, "Device Ports/IDs/Channels"=w203, "Device Engine Path"=w204) -> ("Notifier Name"=w194:string)  [unwired: 11 in, 1 out]
      n67 = call "Device Launcher.vi"("Notifier Name"=w200, "Device Ports/IDs/Channels"=w202, "Device Engine Path"=w201) -> ("Notifier Name"=w193:string)  [unwired: 11 in, 1 out]
      n68 = while {
        tunnel: [FALSE] -> w208
        tunnel: w196 -> [w1148]
        tunnel: w195 -> [w1147]
        tunnel: w194 -> [w1146]
        tunnel: w193 -> [w1145]
        stop <- w1150 stop-if-true
        n69 = event shown="[9] \"Start Lock\": Value Change" {
          selector: _ -> [_ _ _ _ _ _ _ _ _ _ _ _]
          dyn-events: _ -> [_ _ _ _ _ _ _ _ _ _ _ _]
          timeout: -1 -> [_ _ _ _ _ _ _ _ _ _ _ _]
          tunnel: FALSE -> [w1153 w1157 w1160 w1170 w1190 w1225 w1252 w1259 w1288 w1298 w1305 _]
          tunnel: [w1153 w1157 w1160 w1170 w1190 w1225 w1252 w1259 w1288 w1298 w1305 w1315] -> w1150
          tunnel: w1148 -> [_ _ w1159 _ _ _ _ _ _ _ _ _]
          tunnel: w1147 -> [_ _ _ w1169 w1187 w1228 w1251 w1258 w1287 w1297 w1304 w1310]
          tunnel: w1146 -> [_ _ _ _ _ _ _ _ _ _ _ _]
          tunnel: w1145 -> [_ _ _ _ _ _ _ _ _ _ _ _]
          event Timeout {
            n70 = event-data() -> ()  [unwired: 1 in, 1 out]
          }
          event Application Instance Close? {
            n71 = event-data() -> ()  [unwired: 1 in, 1 out]
            n72 = control-ref of="This VI"() -> (w1154:refnum<vi>)
            n73 = invoke class="VI" method="FP.Open"(reference=w1154, "Activate"=TRUE ("Activate?"), "State"=T16."Standard") -> ()  [unwired: 2 in, 5 out]
            n74 = event-data("Discard?"=TRUE) -> ()  [unwired: 1 in, 1 out]
          }
          event "Set Camera ROI": Value Change {
            n75 = event-data() -> ()  [unwired: 1 in, 2 out]
            n76 = call "4Pi Obj Lock - Setup Camera.vi"("Camera Notifier Name"=w1159) -> ()  [unwired: 14 in, 1 out]
          }
          event "XY Correction Active", "Z Correction Active", "Abort If Error": Value Change {
            n77 = event-data() -> ("NewVal"=w1165:bool, "CtlRef"=w1168:refnum<vi>)  [unwired: 1 in]
            n78 = Get Notifier Status(notifier=w1169) -> (notifier out=w1167:refnum<notifier>, current notification=w1164:T8)  [unwired: 1 in, 3 out]
            n79 = property class="Bool (strict)"(reference=w1168) -> ("Label.Text"=w1166:string)  [unwired: 1 in, 2 out]
            n80 = case shown="\"XY Correction Active\"" w1166 {
              tunnel: w1165 -> [_ w1173 w1176 w1179]
              tunnel: w1164 -> [w1171 w1174 w1177 w1180]
              tunnel: [w1171 w1172 w1175 w1178] -> w1163
              frame Default {
              }
              frame "XY Correction Active" {
                n81 = Bundle By Name(cluster=w1174, "XY Correction Active"=w1173) -> (w1172:T8)
              }
              frame "Z Correction Active" {
                n82 = Bundle By Name(cluster=w1177, "Z Correction Active"=w1176) -> (w1175:T8)
              }
              frame "Abort If Error" {
                n83 = Bundle By Name(cluster=w1180, "Abort If Error"=w1179) -> (w1178:T8)
              }
            }
            n84 = Bundle By Name(cluster=w1163, "Actions"=4Pi_Obj_Lock_-_Actions."Idle") -> (w1161:T8)
            n85 = Send Notification(notification=w1161, notifier=w1167) -> ()  [unwired: 1 in, 2 out]
          }
          event "Z Drift Threshold", "Z Stage Move Limit (µm)", "XY Drift Threshold", "XY Stage Move Limit (µm)", "P (Proportional)", "I (Integral)", "D (Derivative)", "Sample Z Step Size (µm)": Value Change {
            n86 = event-data() -> ("NewVal"=w1185:dbl, "CtlRef"=w1186:refnum<vi>)  [unwired: 1 in]
            n87 = Get Notifier Status(notifier=w1187) -> (notifier out=w1184:refnum<notifier>, current notification=w1188:T8)  [unwired: 1 in, 3 out]
            n88 = property class="DigNum (strict)"(reference=w1186) -> ("Label.Text"=w1189:string)  [unwired: 1 in, 2 out]
            n89 = case shown="\"Sample Z Step Size (µm)\"" w1189 {
              tunnel: w1185 -> [_ w1193 w1196 w1199 w1202 w1207 w1213 w1219 w1223]
              tunnel: w1188 -> [w1191 w1194 w1197 w1200 w1203 w1206 w1212 w1218 w1224]
              tunnel: [w1191 w1192 w1195 w1198 w1201 w1204 w1210 w1216 w1222] -> w1182
              frame Default {
              }
              frame "Z Drift Threshold" {
                n90 = Bundle By Name(cluster=w1194, "Z Drift Threshold"=w1193) -> (w1192:T8)
              }
              frame "Z Stage Move Limit (µm)" {
                n91 = Bundle By Name(cluster=w1197, "Z Stage Move Limit (µm)"=w1196) -> (w1195:T8)
              }
              frame "XY Drift Threshold" {
                n92 = Bundle By Name(cluster=w1200, "XY Drift Threshold"=w1199) -> (w1198:T8)
              }
              frame "XY Stage Move Limit (µm)" {
                n93 = Bundle By Name(cluster=w1203, "XY Stage Move Limit (µm)"=w1202) -> (w1201:T8)
              }
              frame "P (Proportional)" {
                n94 = Unbundle By Name(w1206) -> ("PID Values"=w1209:dbl[])
                n95 = Replace Array Subset(array=w1209, new element=w1207, index=0) -> (w1205:dbl[])
                n96 = Bundle By Name(cluster=w1206, "PID Values"=w1205) -> (w1204:T8)
              }
              frame "I (Integral)" {
                n97 = Unbundle By Name(w1212) -> ("PID Values"=w1215:dbl[])
                n98 = Replace Array Subset(array=w1215, new element=w1213, index=1) -> (w1211:dbl[])
                n99 = Bundle By Name(cluster=w1212, "PID Values"=w1211) -> (w1210:T8)
              }
              frame "D (Derivative)" {
                n100 = Unbundle By Name(w1218) -> ("PID Values"=w1221:dbl[])
                n101 = Replace Array Subset(array=w1221, new element=w1219, index=2) -> (w1217:dbl[])
                n102 = Bundle By Name(cluster=w1218, "PID Values"=w1217) -> (w1216:T8)
              }
              frame "Sample Z Step Size (µm)" {
                n103 = Bundle By Name(cluster=w1224, "Z Step Size (µm)"=w1223) -> (w1222:T8)
              }
            }
            n104 = Bundle By Name(cluster=w1182, "Actions"=4Pi_Obj_Lock_-_Actions."Idle") -> (w1181:T8)
            n105 = Send Notification(notification=w1181, notifier=w1184) -> ()  [unwired: 1 in, 2 out]
          }
          event "Sample Z Step No.": Value Change {
            n106 = event-data() -> ("NewVal"=w1226:u32)  [unwired: 1 in]
            n107 = for {
              N: w1226 -> [_]
              tunnel: [w1245] -> w1230 mode=indexing
              tunnel: [w1234] -> w1229 mode=indexing
              i -> [w1244]
              w1235 = T12 3 items=["Grayscale (U8)", "Grayscale (I16)", "Grayscale (SGL)", "Complex (CSG)", "RGB (U32)", "HSL (U32)", "RGB (U64)", "Grayscale (U16)"] ("Image Type")
              w1240 = T12 2 items=["Grayscale (U8)", "Grayscale (I16)", "Grayscale (SGL)", "Complex (CSG)", "RGB (U32)", "HSL (U32)", "RGB (U64)", "Grayscale (U16)"] ("Image Type")
              w1236 = 10 ("Border Size")
              n108 = Number To Decimal String(number=w1244, width (-)=i16 1) -> (decimal integer string=w1242:string)
              n109 = Concatenate Strings("Ref Stack " ("string"), w1242) -> (w1238:string)
              n110 = call "IMAQ Create"("Border Size"=w1236, "Image Name"=w1238, "Image Type"=w1240) -> ("New Image"=w1245:T9)  [unwired: 2 in, 1 out]
              n111 = Concatenate Strings("FFT" ("string"), w1238) -> (w1237:string)
              n112 = call "IMAQ Create"("Border Size"=w1236, "Image Name"=w1237, "Image Type"=w1235) -> ("New Image"=w1234:T9)  [unwired: 2 in, 1 out]
            }
            n113 = Get Notifier Status(notifier=w1228) -> (notifier out=w1232:refnum<notifier>, current notification=w1233:T8)  [unwired: 1 in, 3 out]
            n114 = Bundle By Name(cluster=w1233, "Actions"=4Pi_Obj_Lock_-_Actions."Idle", "Z Step No."=w1226, "Ref Stack (SGL)"=w1230, "Ref FFT Stack (CSG)"=w1229) -> (w1231:T8)
            n115 = Send Notification(notification=w1231, notifier=w1232) -> ()  [unwired: 1 in, 2 out]
          }
          event "Frame Accumulations": Value Change {
            n116 = event-data() -> ("NewVal"=w1248:u16)  [unwired: 1 in]
            n117 = Get Notifier Status(notifier=w1251) -> (notifier out=w1250:refnum<notifier>, current notification=w1249:T8)  [unwired: 1 in, 3 out]
            n118 = Bundle By Name(cluster=w1249, "Actions"=4Pi_Obj_Lock_-_Actions."Idle", "Frame Accumulations"=w1248) -> (w1247:T8)
            n119 = Send Notification(notification=w1247, notifier=w1250) -> ()  [unwired: 1 in, 2 out]
          }
          event "Update Delay (ms)": Value Change {
            n120 = event-data() -> ("NewVal"=w1255:i32)  [unwired: 1 in]
            n121 = Get Notifier Status(notifier=w1258) -> (notifier out=w1257:refnum<notifier>, current notification=w1256:T8)  [unwired: 1 in, 3 out]
            n122 = Bundle By Name(cluster=w1256, "Actions"=4Pi_Obj_Lock_-_Actions."Idle", "Update Delay (ms)"=w1255) -> (w1254:T8)
            n123 = Send Notification(notification=w1254, notifier=w1257) -> ()  [unwired: 1 in, 2 out]
          }
          event "Save Lock Settings": Value Change {
            n124 = event-data() -> ()  [unwired: 1 in, 1 out]
            n125 = Wait on Notification(notifier=w1287) -> (notification=w1285:T8)  [unwired: 3 in, 3 out]
            n126 = Unbundle By Name(w1285) -> ("Z Step Size (µm)"=w1261:dbl, "Z Step No."=w1260:u32, "Z Drift Threshold"=w1284:dbl, "Z Stage Move Limit (µm)"=w1283:dbl, "XY Drift Threshold"=w1282:dbl, "XY Stage Move Limit (µm)"=w1281:dbl, "Frame Accumulations"=w1280:u16, "Abort If Error"=w1279:bool, "Z Correction Active"=w1278:bool, "XY Correction Active"=w1277:bool, "PID Values"=w1267:dbl[])
            n127 = local read "Invert X Axis"() -> (w1265:bool)
            n128 = local read "Invert Y Axis"() -> (w1264:bool)
            n129 = local read "Invert Z Axis"() -> (w1263:bool)
            n130 = local read "Flip XY Axis"() -> (w1266:bool)
            n131 = Bundle By Name(cluster=T7 {"Z Drift Threshold"=0.05, "Z Stage Move Limit (µm)"=1.0, "XY Drift Threshold"=0.05, "XY Stage Move Limit (µm)"=1.0, "Frame Accumulations"=10, "Abort If Error"=FALSE, "Flip XY Axis"=FALSE, "Invert X Axis"=FALSE, "Invert Y Axis"=FALSE, "Invert Z Axis"=FALSE, "Z Correction Active"=TRUE, "XY Correction Active"=TRUE, "PID Values"=[], "Update Delay (ms)"=0, "Sample Z Step Size (µm)"=2.0, "Sample Z Step No."=2, "Z Update Scale Factor"=2.0, "Y Update Scale Factor"=2.0, "X Update Scale Factor"=2.0} ("Lock Settings"), "Sample Z Step Size (µm)"=w1261, "Sample Z Step No."=w1260, "Z Drift Threshold"=w1284, "Z Stage Move Limit (µm)"=w1283, "XY Drift Threshold"=w1282, "XY Stage Move Limit (µm)"=w1281, "Frame Accumulations"=w1280, "Abort If Error"=w1279, "Z Correction Active"=w1278, "XY Correction Active"=w1277, "PID Values"=w1267, "Flip XY Axis"=w1266, "Invert X Axis"=w1265, "Invert Y Axis"=w1264, "Invert Z Axis"=w1263) -> (w1276:T7)
            n132 = control-ref of="This VI"() -> (w1274:refnum<vi>)
            n133 = Flatten To JSON(anything=w1276) -> (JSON string=w1269:string)  [unwired: 2 in, 1 out]
            n134 = property class="VI"(reference=w1274) -> ("Path"=w1271:path)  [unwired: 1 in, 2 out]
            n135 = Strip Path(path=w1271) -> (stripped path=w1270:path)  [unwired: 1 out]
            n136 = Build Path(base path=w1270, name or relative path="4Pi Objective Lock Default Settings") -> (appended path=w1272:path)
            n137 = Build Path(base path=w1272, name or relative path="Default Obj Lock Settings.json") -> (appended path=w1268:path)
            n138 = Write to Text File(file (use dialog)=w1268, text=w1269) -> (refnum out=w1262:refnum<file>)  [unwired: 2 in, 2 out]
            n139 = Close File(refnum=w1262) -> ()  [unwired: 1 in, 2 out]
          }
          event "Start Lock": Value Change {
            n140 = event-data() -> ("NewVal"=w1294:bool)  [unwired: 1 in]
            n141 = Select(t=4Pi_Obj_Lock_-_Actions."Start Lock", s=w1294, f=4Pi_Obj_Lock_-_Actions."Abort" ("Actions")) -> (s? t:f=w1292:T6)
            n142 = Get Notifier Status(notifier=w1297) -> (notifier out=w1296:refnum<notifier>, current notification=w1295:T8)  [unwired: 1 in, 3 out]
            n143 = Bundle By Name(cluster=w1295, "Actions"=w1292, "Running?"=TRUE) -> (w1291:T8)
            n144 = Send Notification(notification=w1291, notifier=w1296) -> ()  [unwired: 1 in, 2 out]
          }
          event "Restart Lock": Value Change {
            n145 = event-data() -> ()  [unwired: 1 in, 1 out]
            n146 = Get Notifier Status(notifier=w1304) -> (notifier out=w1303:refnum<notifier>, current notification=w1302:T8)  [unwired: 1 in, 3 out]
            n147 = Bundle By Name(cluster=w1302, "Actions"=4Pi_Obj_Lock_-_Actions."Restart Lock" ("t")) -> (w1301:T8)
            n148 = local write "Start Lock"(TRUE ("Start Lock")) -> ()
            n149 = Send Notification(notification=w1301, notifier=w1303) -> ()  [unwired: 1 in, 2 out]
          }
          event "Quit": Value Change {
            # "Turn off the OBJ lock before quiting."
            n150 = event-data() -> ("NewVal"=w1315:bool)  [unwired: 1 in]
            n151 = Get Notifier Status(notifier=w1310) -> (notifier out=w1308:refnum<notifier>, current notification=w1306:T8)  [unwired: 1 in, 3 out]
            n152 = Unbundle By Name(w1306) -> ("Running?"=w1309:bool)
            n153 = case shown="True" w1309 {
              tunnel: w1308 -> [w1316 w1320]
              tunnel: [w1316 w1317] -> w1307
              tunnel: w1306 -> [_ w1322]
              frame False {
              }
              frame True {
                n154 = Bundle By Name(cluster=w1322, "Actions"=4Pi_Obj_Lock_-_Actions."Abort") -> (w1319:T8)
                n155 = Send Notification(notification=w1319, notifier=w1320) -> (notifier out=w1318:refnum<notifier>)  [unwired: 1 in, 1 out]
                n156 = while {
                  tunnel: w1318 -> [w1332]
                  tunnel: [w1327] -> w1317
                  i -> [w1326]
                  stop <- w1328 stop-if-true
                  n157 = Get Notifier Status(notifier=w1332) -> (notifier out=w1327:refnum<notifier>, # waiting=w1331:i32)  [unwired: 1 in, 3 out]
                  n158 = Greater?(x=w1326, y=1500) -> (0:w1324:bool)
                  n159 = Less?(x=w1331, y=1) -> (x < y?=w1329:bool)
                  n160 = Or(x=w1329, y=w1324) -> (x .or. y?=w1328:bool)
                  n161 = Wait (ms)(milliseconds to wait=u32 1) -> ()  [unwired: 1 out]
                }
              }
            }
            n162 = Get Notifier Status(notifier=w1307) -> (notifier out=w1312:refnum<notifier>, current notification=w1314:T8)  [unwired: 1 in, 3 out]
            n163 = Bundle By Name(cluster=w1314, "Actions"=4Pi_Obj_Lock_-_Actions."Quit") -> (w1311:T8)
            n164 = Send Notification(notification=w1311, notifier=w1312) -> ()  [unwired: 1 in, 2 out]
          }
        }
      }
      n165 = while {
        tunnel: w196 -> [w222]
        tunnel: w194 -> [w210]
        tunnel: w193 -> [w209]
        tunnel: w195 -> [w221]
        stop <- w217 stop-if-true
        # "Column 1 - Target Lock Values\nColumn 2 - Current Values\nColumn 3 - Differnce Values\nColumn 4 - Initial XYZ Stage Positions"
        n166 = Wait on Notification(notifier=w221, ignore previous (F)=FALSE) -> (notifier out=w216:refnum<notifier>, notification=w219:T8)  [unwired: 2 in, 2 out]
        n167 = Unbundle By Name(w219) -> ("Actions"=w211:T6)
        n168 = Equal?(x=4Pi_Obj_Lock_-_Actions."Quit", y=w211) -> (x = y?=w217:bool)
        n169 = Initialize Array(0.0 ("element"), 3 ("dimension size"), 4 ("dimension size")) -> (w213:dbl[][])
        n170 = while {
          shift-right: [w229] -> _
          shift-left: w211 -> [w237]
          tunnel: w222 -> [w241]
          tunnel: w210 -> [w240]
          tunnel: w209 -> [w239]
          tunnel: w216 -> [w235]
          shift-right: [w223] -> _
          shift-left: w213 -> [w224]
          stop <- w236 stop-if-true
          w231 = 4Pi_Obj_Lock_-_Actions."Abort" ("x")
          n171 = case shown="\"Move Z\"" w237 {
            tunnel: w241 -> [_ w261 _ w366 _ _ w476 w510 w553 w599 _ w664 _ _ _ _ _ _ _ _ w1114 _ _]
            tunnel: w240 -> [_ w294 _ _ _ _ w452 _ _ _ _ _ _ w757 _ w848 w897 _ _ _ _ _ _]
            tunnel: w239 -> [_ w293 w322 w367 _ w427 w451 _ _ _ _ _ _ w756 w817 _ _ w973 _ _ _ _ _]
            tunnel: FALSE -> [w244 w306 w318 w365 w405 w423 w479 w541 w555 w601 w637 w694 w739 w763 w822 w851 w923 w978 w1089 w1101 w1118 _ _]
            tunnel: [4Pi_Obj_Lock_-_Actions."Exit Loop" ("x") w263 4Pi_Obj_Lock_-_Actions."Get Ref Stack" ("x") w370 4Pi_Obj_Lock_-_Actions."Move To Init Z" ("x") 4Pi_Obj_Lock_-_Actions."Get Current Image" ("x") w471 w524 w558 w604 4Pi_Obj_Lock_-_Actions."Check Drift cc xy" ("x") w681 w717 w767 w825 w854 w912 w954 4Pi_Obj_Lock_-_Actions."Delay" ("x") 4Pi_Obj_Lock_-_Actions."Get Current Image" ("x") 4Pi_Obj_Lock_-_Actions."Exit Loop" ("x") 4Pi_Obj_Lock_-_Actions."Exit Loop" ("x") 4Pi_Obj_Lock_-_Actions."Quit" ("x")] -> w230
            tunnel: [w244 w306 w318 w365 w405 w423 w479 w541 w555 w601 w637 w694 w739 w763 w822 w851 w923 w978 w1089 w1101 w1118 TRUE TRUE] -> w236
            tunnel: w235 -> [w243 w277 w323 w369 w410 w421 w478 w540 w565 w611 w659 w693 w738 w798 w836 w870 w922 w976 w1087 w1099 w1122 w1128 w1132]
            tunnel: [w243 w272 w321 w368 w407 w421 w478 w532 w564 w610 w635 w692 w737 w766 w824 w853 w921 w975 w1086 w1095 w1121 w1128 w1131] -> w234
            tunnel: w224 -> [w242 w290 w317 w364 w404 w422 w464 w539 w554 w600 w636 w669 w727 w762 w821 w850 w889 w952 w1068 w1098 w1117 w1127 w1140]
            tunnel: [w242 w289 w317 w364 w404 w422 w463 w538 w554 w600 w636 w668 w724 w762 w821 w850 w889 w952 w1068 w1098 w1117 w1127 w1140] -> w223
            frame "Idle", Default {
            }
            frame "Start Lock" {
              w256 = T17 [] ("History Data")
              w286 = FALSE ("Move Limit Error")
              w291 = Stage_Actions."Get Position" ("Actions")
              n172 = control-ref of="This VI"() -> (w304:refnum<vi>)
              n173 = call "Stages Messenger.vi"("Stage Notifier Name"=w294, "Actions"=w291) -> ("Positions"=w295:dbl[])  [unwired: 10 in, 3 out]
              n174 = call "Stages Messenger.vi"("Stage Notifier Name"=w293, "Actions"=w291) -> ("Positions"=w296:dbl[])  [unwired: 10 in, 3 out]
              n175 = property class="VI"(reference=w304) -> ("Path"=w301:path)  [unwired: 1 in, 2 out]
              n176 = local write "Move Limit Error"(w286) -> ()
              n177 = local write "Fit Error"(w286) -> ()
              n178 = Index Array(array=w296, index=0) -> (element=w292:dbl)
              n179 = Strip Path(path=w301) -> (stripped path=w300:path)  [unwired: 1 out]
              n180 = Build Path(base path=w300, name or relative path="4Pi Objective Lock Default Settings") -> (appended path=w302:path)
              n181 = Build Array (concatenate)(w295, w292) -> (w271:dbl[])
              n182 = Build Path(base path=w302, name or relative path="Initial Stage Positions.json") -> (appended path=w298:path)
              n183 = Flatten To JSON(anything=w271) -> (JSON string=w299:string)  [unwired: 2 in, 1 out]
              n184 = Replace Array Subset(array=w290, new element=w271, index (col)=3 ("disabled index (col)")) -> (w289:dbl[][])  [unwired: 1 in]
              n185 = Index Array(array=w271, index #1=0 ("index"), index #2=1 ("index"), index #3=2 ("index")) -> (element #1=w267:dbl, element #2=w265:dbl, element #3=w266:dbl)
              n186 = Write to Text File(file (use dialog)=w298, text=w299) -> (refnum out=w287:refnum<file>)  [unwired: 2 in, 2 out]
              n187 = local write "X Axis Position (µm)"(w267) -> ()
              n188 = local write "Y Axis Position (µm)"(w265) -> ()
              n189 = local write "Z Axis Position (µm)"(w266) -> ()
              n190 = Get Notifier Status(notifier=w277) -> (notifier out=w272:refnum<notifier>, current notification=w276:T8)  [unwired: 1 in, 3 out]
              n191 = Close File(refnum=w287) -> ()  [unwired: 1 in, 2 out]
              n192 = Unbundle By Name(w276) -> ("Cur Image (SGL)"=w275:T9)
              n193 = Unbundle By Name(w276) -> ("Z Step No."=w274:u32, "Ref Stack (SGL)"=w273:T9[])
              n194 = call "Camera Messenger.vi"("Notifier Name"=w261, "General Camera Actions"=Generic_Camera_Actions."Get ROI", "Camera ROI"=T14 {"H_Offset"=0, "V_Offset"=0, "H_Width"=0, "V_Width"=0} ("General Camera ROI")) -> ("Notifier Name Dup"=w258:string, "Camera ROI"=w278:T14)  [unwired: 7 in, 4 out]
              n195 = Unbundle By Name(w278) -> ("H_Width"=w283:u16, "V_Width"=w281:u16)
              n196 = To Long Integer(number=w283) -> (32bit integer=w282:i32)
              n197 = To Long Integer(number=w281) -> (32bit integer=w280:i32)
              n198 = Initialize Array(sgl 0.0 ("element"), w282, w280) -> (w246:sgl[][])
              n199 = for {
                N: w274 -> [_]
                tunnel: w246 -> [w315]
                tunnel: w273 -> [w316] mode=indexing
                n200 = call "IMAQ ArrayToImage"("Image Pixels (Float)"=w315, "Image"=w316) -> ()  [unwired: 8 in, 2 out]
              }
              n201 = call "IMAQ ArrayToImage"("Image Pixels (Float)"=w246, "Image"=w275) -> ()  [unwired: 8 in, 2 out]
              n202 = Array Size(array=w246) -> (size(s)=w252:i32[])
              n203 = To Double Precision Float(number=w252) -> (double precision float=w255:dbl[])
              n204 = call "Camera Messenger.vi"("Notifier Name"=w258, "General Camera Actions"=Generic_Camera_Actions."Live Preview") -> ("Notifier Name Dup"=w259:string)  [unwired: 8 in, 5 out]
              n205 = Divide(x=w255, y=2.0 ("index")) -> (x/y=w253:dbl[])
              n206 = while {
                tunnel: w259 -> [w313]
                tunnel: [w308] -> w257
                i -> [w312]
                stop <- w309 stop-if-true
                n207 = call "Camera Messenger.vi"("Notifier Name"=w313, "General Camera Actions"=Generic_Camera_Actions."Status") -> ("Running?"=w310:bool)  [unwired: 8 in, 5 out]
                n208 = Greater?(x=w312, y=3000) -> (0:w308:bool)
                n209 = Or(x=w310, y=w308) -> (x .or. y?=w309:bool)
                n210 = Wait (ms)(milliseconds to wait=u32 1) -> ()  [unwired: 1 out]
              }
              n211 = Round Toward -Infinity(1:w253) -> (0:w251:dbl[])
              n212 = Index Array(array=w251, index #1=0 ("index"), index #2=1 ("index")) -> (element #1=→"Target Y Position cc (px)":dbl, element #2=→"Target X Position cc (px)":dbl)
              n213 = Select(t=4Pi_Obj_Lock_-_Actions."Exit Loop", s=w257, f=4Pi_Obj_Lock_-_Actions."Get Target Z Position" ("x")) -> (s? t:f=w263:T6)
              n214 = property on="X Target and Fit Position (µm)" class="WFChart (strict)"("History Data"=w256) -> ()  [unwired: 2 in, 2 out]
              n215 = property on="Y Target and Fit Position (µm)" class="WFChart (strict)"("History Data"=w256) -> ()  [unwired: 2 in, 2 out]
              n216 = property on="Z Target and Fit Value (µm)" class="WFChart (strict)"("History Data"=w256) -> ()  [unwired: 2 in, 2 out]
            }
            frame "Get Target Z Position" {
              w345 = 0.0 ("Target Z (µm)")
              n217 = Get Notifier Status(notifier=w323) -> (notifier out=w343:refnum<notifier>, current notification=w348:T8)  [unwired: 1 in, 3 out]
              n218 = Unbundle By Name(w348) -> ("Z Step No."=w341:u32, "Z Step Size (µm)"=w340:dbl, "Z Stage Move Limit (µm)"=w338:dbl)
              n219 = Unbundle By Name(w348) -> ("Z Step No."=w333:u32, "Z Step Size (µm)"=w346:dbl)
              n220 = Divide(x=w341, y=2.0) -> (x/y=w331:dbl)
              n221 = Round Toward -Infinity(1:w331) -> (0:w330:dbl)
              n222 = Multiply(x=w330, y=w340) -> (x*y=w335:dbl)
              n223 = Decrement(x=w333) -> (x-1=w332:u32)
              n224 = Negate(x=w335) -> (-x=w334:dbl)
              n225 = Negate(x=w338) -> (-x=w339:dbl)
              n226 = In Range and Coerce(upper limit=w338, x=w334, lower limit=w339) -> (coerced(x)=w336:dbl)  [unwired: 1 out]
              n227 = Add(x=w345, y=w336) -> (x+y=w337:dbl)
              n228 = Build Array(w337) -> (w347:dbl[])
              n229 = for {
                N: w332 -> [_]
                tunnel: w346 -> [w359]
                shift-right: [w360] -> w344
                shift-left: w347 -> [w361]
                shift-right: [w357] -> _
                shift-left: w337 -> [w358]
                n230 = Add(x=w358, y=w359) -> (x+y=w357:dbl)
                n231 = Build Array (concatenate)(w361, w357) -> (w360:dbl[])
              }
              n232 = Build Array(w336) -> (w349:dbl[])
              n233 = call "Stages Messenger.vi"("Stage Notifier Name"=w322, "Actions"=Stage_Actions."MVR", "Setpoint"=w349, "Axis"=bool[] [TRUE], "Exit While Busy?"=TRUE) -> ("Stage Notifier Name (Dup)"=w328:string, "Status"=w329:T18)  [unwired: 7 in, 2 out]
              n234 = case shown="Default" w329 {
                tunnel: [w355] -> w327
                tunnel: w328 -> [w355]
                frame Default {
                  n235 = Wait (ms)(milliseconds to wait=u32 250) -> ()  [unwired: 1 out]
                }
              }
              n236 = Bundle By Name(cluster=w348, "Sample Z (µm)"=w344) -> (w342:T8)
              n237 = call "Stages Messenger.vi"("Stage Notifier Name"=w327, "Actions"=Stage_Actions."Get Position", "Exit While Busy?"=TRUE) -> ("Positions"=w325:dbl[])  [unwired: 9 in, 3 out]
              n238 = Index Array(array=w325, index=0) -> (element=w319:dbl)
              n239 = Send Notification(notification=w342, notifier=w343) -> (notifier out=w321:refnum<notifier>)  [unwired: 1 in, 1 out]
              n240 = local write "Z Axis Position (µm)"(w319) -> ()
              "Target Z (µm)" <- w345
            }
            frame "Get Ref Stack" {
              n241 = Get Notifier Status(notifier=w369) -> (notifier out=w368:refnum<notifier>, current notification=w363:T8)  [unwired: 1 in, 3 out]
              n242 = Unbundle By Name(w363) -> ("Z Step No."=w373:u32, "Ref Stack (SGL)"=w372:T9[])
              n243 = Unbundle By Name(w363) -> ("Frame Accumulations"=w362:u16)
              n244 = Unbundle By Name(w363) -> ("Z Step Size (µm)"=w371:dbl)
              n245 = while {
                tunnel: w366 -> [w391]
                tunnel: w373 -> [w388]
                tunnel: w368 -> [w390]
                tunnel: [w380] -> w370
                tunnel: w372 -> [w379] mode=indexing
                tunnel: w371 -> [w378]
                tunnel: w367 -> [w377]
                tunnel: w362 -> [w374]
                i -> [w387]
                stop <- w383 stop-if-true
                n246 = flat-sequence {
                  tunnel: w391 -> [w394]
                  tunnel: w379 -> [w392]
                  tunnel: w374 -> [w393]
                  tunnel: w378 -> [w398]
                  tunnel: w377 -> [w397]
                  frame #0 {
                    n247 = call "Generic Camera Get New Camera Image.vi"("Camera Notifier Name"=w394, "Frames"=w393) -> ("Image - U16"=w396:u16[][])  [unwired: 11 in, 2 out]
                    n248 = To Single Precision Float(number=w396) -> (single precision float=w395:sgl[][])
                    n249 = call "IMAQ ArrayToImage"("Image Pixels (Float)"=w395, "Image"=w392) -> ()  [unwired: 8 in, 2 out]
                  }
                  frame #1 {
                    n250 = Build Array(w398) -> (w402:dbl[])
                    n251 = Wait (ms)(milliseconds to wait=u32 250) -> ()  [unwired: 1 out]
                    n252 = call "Stages Messenger.vi"("Stage Notifier Name"=w397, "Actions"=Stage_Actions."MVR", "Setpoint"=w402, "Axis"=bool[] [TRUE], "Exit While Busy?"=TRUE) -> ()  [unwired: 7 in, 4 out]
                  }
                }
                n253 = Get Notifier Status(notifier=w390) -> (current notification=w382:T8)  [unwired: 1 in, 4 out]
                n254 = To Unsigned Long Integer(number=w387) -> (unsigned 32bit integer=w386:u32)
                n255 = Increment(x=w386) -> (x+1=w389:u32)
                n256 = Unbundle By Name(w382) -> ("Running?"=w385:bool)
                n257 = Greater Or Equal?(x=w389, y=w388) -> (x >= y?=w384:bool)
                n258 = Not(x=w385) -> (.not. x?=w381:bool)
                n259 = Or(x=w381, y=w384) -> (x .or. y?=w383:bool)
                n260 = Select(t=4Pi_Obj_Lock_-_Actions."Abort" ("x"), s=w381, f=4Pi_Obj_Lock_-_Actions."Cal Ref FFT") -> (s? t:f=w380:T6)
              }
            }
            frame "Cal Ref FFT" {
              n261 = Get Notifier Status(notifier=w410) -> (notifier out=w407:refnum<notifier>, current notification=w411:T8)  [unwired: 1 in, 3 out]
              n262 = Unbundle By Name(w411) -> ("Ref Stack (SGL)"=w409:T9[], "Ref FFT Stack (CSG)"=w408:T9[])
              n263 = for {
                tunnel: w409 -> [w413] mode=indexing
                tunnel: w408 -> [w412] mode=indexing
                n264 = call "4Pi Obj Lock - Norm FFT.vi"("FFT Image Dst"=w412, "Image In"=w413) -> ()  [unwired: 8 in, 2 out]
              }
            }
            frame "Move To Init Z" {
              # "initial z stage position"
              n265 = Index Array(array=w422, index (row)=2, index (col)=3 ("disabled index (col)")) -> (element=w424:dbl)
              n266 = flat-sequence {
                tunnel: w427 -> [w437]
                tunnel: [w436] -> w429
                tunnel: w424 -> [w432]
                tunnel: [w430] -> w428
                tunnel: w429 -> [w442]
                tunnel: w428 -> [w441]
                tunnel: [w440] -> w415
                frame #0 {
                  n267 = call "Stages Messenger.vi"("Stage Notifier Name"=w437, "Actions"=Stage_Actions."Get Position") -> ("Stage Notifier Name (Dup)"=w436:string, "Positions"=w434:dbl[])  [unwired: 10 in, 2 out]
                  n268 = Index Array(array=w434, index=0) -> (element=w433:dbl)
                  n269 = Subtract(x=w432, y=w433) -> (x-y=w431:dbl)
                  n270 = Build Array(w431) -> (w430:dbl[])
                }
                frame #1 {
                  n271 = Wait (ms)(milliseconds to wait=u32 250) -> ()  [unwired: 1 out]
                  n272 = call "Stages Messenger.vi"("Stage Notifier Name"=w442, "Actions"=Stage_Actions."MVR", "Setpoint"=w441, "Axis"=bool[] [TRUE], "Exit While Busy?"=TRUE) -> ("Stage Notifier Name (Dup)"=w440:string)  [unwired: 7 in, 3 out]
                }
              }
              n273 = call "Stages Messenger.vi"("Stage Notifier Name"=w415, "Actions"=Stage_Actions."Get Position", "Exit While Busy?"=TRUE) -> ("Positions"=w418:dbl[])  [unwired: 9 in, 3 out]
              n274 = Index Array(array=w418, index=0) -> (element=w416:dbl)
              n275 = local write "Z Axis Position (µm)"(w416) -> ()
            }
            frame "Restart Lock" {
              w446 = T17 [] ("History Data")
              w447 = FALSE ("Move Limit Error")
              # "Make sure the camera is running, if not abort."
              n276 = control-ref of="This VI"() -> (w469:refnum<vi>)
              n277 = call "Camera Messenger.vi"("Notifier Name"=w476, "General Camera Actions"=Generic_Camera_Actions."Live Preview") -> ("Notifier Name Dup"=w475:string)  [unwired: 8 in, 5 out]
              n278 = property class="VI"(reference=w469) -> (error out=w455:errorcluster, "Path"=w466:path)  [unwired: 1 in, 1 out]
              n279 = while {
                tunnel: w475 -> [w505]
                tunnel: [w500] -> w474
                i -> [w504]
                stop <- w501 stop-if-true
                n280 = call "Camera Messenger.vi"("Notifier Name"=w505, "General Camera Actions"=Generic_Camera_Actions."Status") -> ("Running?"=w502:bool)  [unwired: 8 in, 5 out]
                n281 = Greater?(x=w504, y=3000) -> (0:w500:bool)
                n282 = Or(x=w502, y=w500) -> (x .or. y?=w501:bool)
                n283 = Wait (ms)(milliseconds to wait=u32 1) -> ()  [unwired: 1 out]
              }
              n284 = Strip Path(path=w466) -> (stripped path=w465:path)  [unwired: 1 out]
              n285 = Build Path(base path=w465, name or relative path="4Pi Objective Lock Default Settings") -> (appended path=w467:path)
              n286 = Build Path(base path=w467, name or relative path="Initial Stage Positions.json") -> (appended path=w461:path)
              n287 = Read from Text File(file (use dialog)=w461, error in=w455) -> (refnum out=w460:refnum<file>, text=w459:string, error out=w458:errorcluster)  [unwired: 2 in, 1 out]
              n288 = Close File(refnum=w460, error in=w458) -> (error out=w457:errorcluster)  [unwired: 1 out]
              n289 = local write "Move Limit Error"(w447) -> ()
              n290 = local write "Fit Error"(w447) -> ()
              n291 = Unflatten From JSON(JSON string=w459, type and defaults=dbl[] [], error in (no error)=w457) -> (value=w453:dbl[], error out=w454:errorcluster)  [unwired: 4 in]
              n292 = case shown="Error" w454 {
                tunnel: w453 -> [w481 _]
                tunnel: w452 -> [w488 w493]
                tunnel: w451 -> [w487 w492]
                tunnel: [w481 w491] -> w450
                tunnel: u32 150 ("milliseconds to wait") -> [w480 w490]
                tunnel: [w480 w490] -> w448
                frame No Error {
                  w489 = Stage_Actions."MOVE" ("Actions")
                  n293 = Split 1D Array(array=w481, index=2) -> (first subarray=w485:dbl[], second subarray=w484:dbl[])
                  n294 = call "Stages Messenger.vi"("Stage Notifier Name"=w488, "Actions"=w489, "Setpoint"=w485, "Axis"=bool[] [TRUE, TRUE]) -> ()  [unwired: 8 in, 4 out]
                  n295 = call "Stages Messenger.vi"("Stage Notifier Name"=w487, "Actions"=w489, "Setpoint"=w484, "Axis"=bool[] [TRUE]) -> ()  [unwired: 8 in, 4 out]
                }
                frame Error {
                  w494 = Stage_Actions."Get Position" ("Actions")
                  n296 = call "Stages Messenger.vi"("Stage Notifier Name"=w493, "Actions"=w494) -> ("Positions"=w496:dbl[])  [unwired: 10 in, 3 out]
                  n297 = call "Stages Messenger.vi"("Stage Notifier Name"=w492, "Actions"=w494) -> ("Positions"=w497:dbl[])  [unwired: 10 in, 3 out]
                  n298 = Index Array(array=w497, index=0) -> (element=w495:dbl)
                  n299 = Build Array (concatenate)(w496, w495) -> (w491:dbl[])
                }
              }
              n300 = Wait (ms)(milliseconds to wait=w448) -> ()  [unwired: 1 out]
              n301 = Replace Array Subset(array=w464, new element=w450, index (col)=3 ("disabled index (col)")) -> (w463:dbl[][])  [unwired: 1 in]
              n302 = property on="X Target and Fit Position (µm)" class="WFChart (strict)"("History Data"=w446) -> ()  [unwired: 2 in, 2 out]
              n303 = property on="Y Target and Fit Position (µm)" class="WFChart (strict)"("History Data"=w446) -> ()  [unwired: 2 in, 2 out]
              n304 = property on="Z Target and Fit Value (µm)" class="WFChart (strict)"("History Data"=w446) -> ()  [unwired: 2 in, 2 out]
              n305 = Select(t=4Pi_Obj_Lock_-_Actions."Exit Loop" ("x"), s=w474, f=4Pi_Obj_Lock_-_Actions."Get Initial Position" ("x")) -> (s? t:f=w471:T6)
            }
            frame "Get Initial Position" {
              w517 = 0 ("index")
              # "Set target values"
              n306 = Get Notifier Status(notifier=w540) -> (notifier out=w533:refnum<notifier>, current notification=w509:T8)  [unwired: 1 in, 3 out]
              n307 = Unbundle By Name(w509) -> ("Frame Accumulations"=w508:u16)
              n308 = Bundle By Name(cluster=w509, "Running?"=TRUE) -> (w530:T8)
              n309 = Send Notification(notification=w530, notifier=w533) -> (notifier out=w532:refnum<notifier>)  [unwired: 1 in, 1 out]
              n310 = call "Generic Camera Get New Camera Image.vi"("Camera Notifier Name"=w510, "Frames"=w508) -> ("Image - U16"=w507:u16[][])  [unwired: 11 in, 2 out]
              n311 = call "2D Gaussian - Fit Image U16.vi"("Image In (U16)"=w507) -> ("Best Fit Params"=w537:T19, "Error Out"=w523:errorcluster)  [unwired: 13 in]
              n312 = Unbundle By Name(w523) -> ("status"=w522:bool)
              n313 = Cluster To Array(cluster=w537) -> (array=w536:dbl[])
              n314 = local write "Fit Error"(w522) -> ()
              n315 = Array Subset(array=w536, index=1, length=4) -> (w529:dbl[])
              n316 = Index Array(array=w529, index #1=0 ("index"), index #2=1 ("index"), index #3=2 ("index"), index #4=3 ("index")) -> (element #1=w511:dbl, element #2=w512:dbl, element #3=w519:dbl, element #4=w518:dbl)
              "Target X Position (px)" <- w511
              "Target Y Position (px)" <- w512
              n317 = Divide(x=w519, y=w518) -> (x/y=w513:dbl)
              "Target sx/sy" <- w513
              n318 = Replace Array Subset(array=w539, new element #1=w511, index (row) #1=0 ("disabled index (row)"), index (col) #1=w517, new element #2=w512, index (row) #2=1 ("disabled index (row)"), index (col) #2=w517, new element #3=w513, index (row) #3=2 ("disabled index (row)"), index (col) #3=w517) -> (w538:dbl[][])
              n319 = Select(t=4Pi_Obj_Lock_-_Actions."Abort" ("x"), s=w522, f=4Pi_Obj_Lock_-_Actions."Get Current XY Position" ("x")) -> (s? t:f=w524:T6)
            }
            frame "Get Current Z Position" {
              n320 = Get Notifier Status(notifier=w565) -> (notifier out=w564:refnum<notifier>, current notification=w552:T8)  [unwired: 1 in, 3 out]
              n321 = Unbundle By Name(w552) -> ("Ref FFT Stack (CSG)"=w571:T9[])
              n322 = Unbundle By Name(w552) -> ("Cur Image (SGL)"=w548:T9, "Tmp Image FFT (CSG)"=w561:T9[])
              n323 = Unbundle By Name(w552) -> ("CC Image (SGL)"=w543:T9, "CC Image Max (SGL)"=w542:T9)
              n324 = Unbundle By Name(w552) -> ("Sample Z (µm)"=w573:dbl[])
              n325 = Unbundle By Name(w552) -> ("Frame Accumulations"=w551:u16)
              n326 = call "Generic Camera Get New Camera Image.vi"("Camera Notifier Name"=w553, "Frames"=w551) -> ("Image - U16"=w550:u16[][])  [unwired: 11 in, 2 out]
              n327 = Index Array(array=w561, index #1=0 ("index"), index #2=1 ("index"), index #3=2 ("index")) -> (element #1=w559:T9, element #2=w545:T9, element #3=w544:T9)
              n328 = To Single Precision Float(number=w550) -> (single precision float=w547:sgl[][])
              n329 = call "IMAQ ArrayToImage"("Image Pixels (Float)"=w547, "Image"=w548) -> ("Image Out"=w549:T9)  [unwired: 8 in, 1 out]
              n330 = call "4Pi Obj Lock - Norm FFT.vi"("FFT Image Dst"=w559, "Image In"=w549) -> ("FFT Image Out"=w569:T9)  [unwired: 8 in, 1 out]
              n331 = call "IMAQ ComplexConjugate"("Image Src"=w569) -> ("Image Dst Out"=w568:T9)  [unwired: 3 in, 1 out]
              n332 = for {
                tunnel: [w578] -> w574 mode=indexing
                tunnel: w568 -> [w584]
                tunnel: w571 -> [w583] mode=indexing
                shift-right: [w578] -> _
                shift-left: sgl 0.0 ("Max CC") -> [w579]
                tunnel: w545 -> [w582]
                tunnel: w544 -> [w581]
                tunnel: w543 -> [w577]
                tunnel: w542 -> [w575]
                n333 = call "4Pi Obj Lock - Get Cross Correlation.vi"("Ref FFT image"=w583, "Cur FFT Image"=w584, "FFT CC image"=w582, "iFFT image"=w581, "CC image"=w577) -> ("Max CC"=w578:sgl, "CC image Out"=w576:T9)  [unwired: 8 in, 1 out]
                n334 = Greater?(x=w578, y=w579) -> (0:w580:bool)
                n335 = case shown="True" w580 {
                  tunnel: w576 -> [_ w586]
                  tunnel: w575 -> [_ w585]
                  frame False {
                  }
                  frame True {
                    n336 = call "IMAQ Copy"("Image Dst"=w585, "Image Src"=w586) -> ()  [unwired: 4 in, 2 out]
                  }
                }
              }
              n337 = To Double Precision Float(number=w574) -> (double precision float=w570:dbl[])
              n338 = call "4Pi Obj Lock - Find Peak Position.vi"("Fit Size"=2, "y"=w570, "x"=w573) -> ("Coerced Peak Position"=w567:dbl)  [unwired: 7 in, 1 out]
              "Measured Z (µm)" <- w567
              n339 = Not A Number/Path/Refnum?(number/path/refnum=w567) -> (NaN/Path/Refnum?=w566:bool)
              n340 = Select(t=4Pi_Obj_Lock_-_Actions."Get Current Z Position" ("x"), s=w566, f=4Pi_Obj_Lock_-_Actions."Check Drift cc z") -> (s? t:f=w558:T6)
            }
            frame "Get Current Image" {
              n341 = Get Notifier Status(notifier=w611) -> (notifier out=w610:refnum<notifier>, current notification=w598:T8)  [unwired: 1 in, 3 out]
              n342 = Unbundle By Name(w598) -> ("CC Image (SGL)"=w589:T9, "CC Image Max (SGL)"=w588:T9)
              n343 = Unbundle By Name(w598) -> ("Ref FFT Stack (CSG)"=w616:T9[])
              n344 = Unbundle By Name(w598) -> ("Cur Image (SGL)"=w594:T9, "Tmp Image FFT (CSG)"=w607:T9[])
              n345 = Unbundle By Name(w598) -> ("Sample Z (µm)"=w618:dbl[])
              n346 = Unbundle By Name(w598) -> ("Frame Accumulations"=w597:u16)
              n347 = call "Generic Camera Get New Camera Image.vi"("Camera Notifier Name"=w599, "Frames"=w597) -> ("Image - U16"=w596:u16[][])  [unwired: 11 in, 2 out]
              n348 = Index Array(array=w607, index #1=0 ("index"), index #2=1 ("index"), index #3=2 ("index")) -> (element #1=w605:T9, element #2=w591:T9, element #3=w590:T9)
              n349 = To Single Precision Float(number=w596) -> (single precision float=w593:sgl[][])
              n350 = call "IMAQ ArrayToImage"("Image Pixels (Float)"=w593, "Image"=w594) -> ("Image Out"=w595:T9)  [unwired: 8 in, 1 out]
              n351 = call "4Pi Obj Lock - Norm FFT.vi"("FFT Image Dst"=w605, "Image In"=w595) -> ("FFT Image Out"=w614:T9)  [unwired: 8 in, 1 out]
              n352 = call "IMAQ ComplexConjugate"("Image Src"=w614) -> ("Image Dst Out"=w613:T9)  [unwired: 3 in, 1 out]
              n353 = for {
                tunnel: [w623] -> w619 mode=indexing
                tunnel: w613 -> [w629]
                tunnel: w616 -> [w628] mode=indexing
                shift-right: [w623] -> _
                shift-left: sgl 0.0 ("Max CC") -> [w624]
                tunnel: w591 -> [w627]
                tunnel: w590 -> [w626]
                tunnel: w589 -> [w622]
                tunnel: w588 -> [w620]
                n354 = call "4Pi Obj Lock - Get Cross Correlation.vi"("Ref FFT image"=w628, "Cur FFT Image"=w629, "FFT CC image"=w627, "iFFT image"=w626, "CC image"=w622) -> ("Max CC"=w623:sgl, "CC image Out"=w621:T9)  [unwired: 8 in, 1 out]
                n355 = Greater?(x=w623, y=w624) -> (0:w625:bool)
                n356 = case shown="False" w625 {
                  tunnel: w621 -> [_ w631]
                  tunnel: w620 -> [_ w630]
                  frame False {
                  }
                  frame True {
                    n357 = call "IMAQ Copy"("Image Dst"=w630, "Image Src"=w631) -> ()  [unwired: 4 in, 2 out]
                  }
                }
              }
              n358 = To Double Precision Float(number=w619) -> (double precision float=w615:dbl[])
              n359 = call "4Pi Obj Lock - Find Peak Position.vi"("Fit Size"=2, "y"=w615, "x"=w618) -> ("Coerced Peak Position"=w587:dbl)  [unwired: 7 in, 1 out]
              n360 = local write "Measured Z (µm)"(w587) -> ()
              n361 = Not A Number/Path/Refnum?(number/path/refnum=w587) -> (NaN/Path/Refnum?=w612:bool)
              n362 = Select(t=4Pi_Obj_Lock_-_Actions."Get Current Image" ("x"), s=w612, f=4Pi_Obj_Lock_-_Actions."Get Current XY Position") -> (s? t:f=w604:T6)
            }
            frame "Get Current XY Position" {
              w647 = 3 ("edge size")
              n363 = Get Notifier Status(notifier=w659) -> (notifier out=w635:refnum<notifier>, current notification=w658:T8)  [unwired: 1 in, 3 out]
              n364 = Unbundle By Name(w658) -> ("CC Image Max (SGL)"=w657:T9)
              n365 = call "IMAQ ImageToArray"("Image"=w657) -> ("Image Pixels (Float)"=w644:sgl[][])  [unwired: 3 in, 4 out]
              n366 = call "4Pi Obj Lock - FFT shift 2D.vi"("Input image"=w644) -> ("fft shifted image"=w643:sgl[][])  [unwired: 10 in]
              n367 = call "4Pi Obj Lock - Crop Imag at Max.vi"("edge size"=w647, "Input array"=w643) -> ("Y"=w653:i32, "X"=w654:i32, "subarray"=w656:sgl[][])  [unwired: 6 in, 1 out]
              n368 = To Double Precision Float(number=w656) -> (double precision float=w633:dbl[][])
              n369 = Build Array(w654, w653) -> (w652:i32[])
              n370 = call "2D Gaussian - Fit -init.vi"("Image In (DBL)"=w633, "width"=10.0) -> ("Best Fit Params"=w655:T19)  [unwired: 12 in, 1 out]
              n371 = To Double Precision Float(number=w652) -> (double precision float=w649:dbl[])
              n372 = Unbundle By Name(w655) -> ("X Position"=w651:dbl, "Y Position"=w650:dbl)
              n373 = Build Array(w651, w650) -> (w648:dbl[])
              n374 = To Double Precision Float(number=w647) -> (double precision float=w646:dbl)
              n375 = Subtract(x=w648, y=w646) -> (x-y=w645:dbl[])
              n376 = Add(x=w645, y=w649) -> (x+y=w640:dbl[])
              n377 = Index Array(array=w640, index #1=0 ("index"), index #2=1 ("index")) -> (element #1=→"Measured X Position cc (px)":dbl, element #2=→"Measured Y Position cc (px)":dbl)
            }
            frame "Get Current Position" {
              w673 = 1 ("index")
              # "retake current image"
              # "Update current values"
              n378 = Get Notifier Status(notifier=w693) -> (notifier out=w692:refnum<notifier>, current notification=w661:T8)  [unwired: 1 in, 3 out]
              n379 = Unbundle By Name(w661) -> ("Abort If Error"=w686:bool, "Cur Image (SGL)"=w663:T9)
              n380 = case shown="False" FALSE {
                tunnel: w664 -> [_ w703]
                tunnel: w663 -> [w697 w700]
                tunnel: w661 -> [_ w702]
                tunnel: [w695 w699] -> w660
                frame False {
                  n381 = call "IMAQ ImageToArray"("Image"=w697) -> ("Image Pixels (Float)"=w696:sgl[][])  [unwired: 3 in, 4 out]
                  n382 = To Unsigned Word Integer(number=w696) -> (unsigned 16bit integer=w695:u16[][])
                }
                frame True {
                  n383 = Unbundle By Name(w702) -> ("Frame Accumulations"=w701:u16)
                  n384 = call "Generic Camera Get New Camera Image.vi"("Camera Notifier Name"=w703, "Frames"=w701) -> ("Image - U16"=w699:u16[][])  [unwired: 11 in, 2 out]
                  n385 = To Single Precision Float(number=w699) -> (single precision float=w698:sgl[][])
                  n386 = call "IMAQ ArrayToImage"("Image Pixels (Float)"=w698, "Image"=w700) -> ()  [unwired: 8 in, 2 out]
                }
              }
              n387 = call "2D Gaussian - Fit Image U16.vi"("Image In (U16)"=w660) -> ("Best Fit Params"=w691:T19, "Error Out"=w687:errorcluster)  [unwired: 13 in]
              n388 = Unbundle By Name(w687) -> ("status"=w685:bool)
              "Fit Error" <- w685
              n389 = And(x=w686, y=w685) -> (x .and. y?=w684:bool)
              n390 = Cluster To Array(cluster=w691) -> (array=w690:dbl[])
              n391 = Array Subset(array=w690, index=1, length=4) -> (w674:dbl[])
              n392 = Index Array(array=w674, index #1=0 ("index"), index #2=1 ("index"), index #3=2 ("index"), index #4=3 ("index")) -> (element #1=w665:dbl, element #2=w666:dbl, element #3=w676:dbl, element #4=w675:dbl)
              "Measured X Position (px)" <- w665
              "Measured Y Position (px)" <- w666
              n393 = Divide(x=w676, y=w675) -> (x/y=w667:dbl)
              "Measured sx/sy" <- w667
              n394 = Select(t=4Pi_Obj_Lock_-_Actions."Abort" ("x"), s=w684, f=4Pi_Obj_Lock_-_Actions."Check Drift cc" ("x")) -> (s? t:f=w681:T6)
              n395 = Replace Array Subset(array=w669, new element #1=w665, index (row) #1=0 ("disabled index (row)"), index (col) #1=w673, new element #2=w666, index (row) #2=1 ("disabled index (row)"), index (col) #2=w673, new element #3=w667, index (row) #3=2 ("disabled index (row)"), index (col) #3=w673) -> (w668:dbl[][])
            }
            frame "Check Drift" {
              # "Update the PID difference between target values and current values"
              # "Check if Sigma X / Sigma Y is over the limit"
              # "Check if XY values are over the limit"
              n396 = Get Notifier Status(notifier=w738) -> (notifier out=w737:refnum<notifier>, current notification=w736:T8)  [unwired: 1 in, 3 out]
              n397 = Unbundle By Name(w736) -> ("Z Correction Active"=w713:bool, "XY Correction Active"=w715:bool, "XY Drift Threshold"=w706:dbl, "Z Drift Threshold"=w708:dbl, "PID Values"=w735:dbl[])
              n398 = Index Array(array=w727, index (col) #1=0 ("disabled index (col)"), index (col) #2=1 ("index (col)")) -> (element #1=w729:dbl[], element #2=w728:dbl[])  [unwired: 2 in]
              n399 = Array To Cluster(array=w735) -> (cluster=w709:T20)
              n400 = local read "pixel size (µm)"() -> (w705:dbl)
              n401 = Build Array(w709) -> (w734:T21)
              n402 = Divide(x=w706, y=w705) -> (x/y=w707:dbl)
              n403 = call-poly <vilib>:"PID.vi"("PID gains"=w734, "process variable"=w728, "setpoint"=w729) -> ("output"=w725:dbl[])  [unwired: 7 in, 1 out]
              n404 = Build Array(w707, w707, w708) -> (w732:dbl[])
              n405 = Replace Array Subset(array=w727, new element=w725, index (col)=2 ("disabled index (col)")) -> (w724:dbl[][])  [unwired: 1 in]
              n406 = Absolute Value(x=w725) -> (abs(x)=w733:dbl[])
              n407 = Greater?(x=w733, y=w732) -> (0:w723:bool[])
              n408 = Split 1D Array(array=w723, index=2) -> (first subarray=w721:bool[], second subarray=w720:bool[])
              n409 = Or Array Elements(Boolean array=w721) -> (logical OR=w716:bool)
              n410 = Or Array Elements(Boolean array=w720) -> (logical OR=w704:bool)
              n411 = And(x=w715, y=w716) -> (x .and. y?=w714:bool)
              n412 = And(x=w713, y=w704) -> (x .and. y?=w712:bool)
              n413 = Build Array(w714, w712) -> (w719:bool[])
              n414 = Boolean Array To Number(Boolean array=w719) -> (number=w718:u32)
              n415 = case shown="0, Default" w718 {
                tunnel: [4Pi_Obj_Lock_-_Actions."Update Plots" ("x") 4Pi_Obj_Lock_-_Actions."Move XY" ("x") 4Pi_Obj_Lock_-_Actions."Move Z" ("x") 4Pi_Obj_Lock_-_Actions."Move XYZ" ("x")] -> w717
                tunnel: [w740 TRUE FALSE w748] -> w711
                tunnel: [w740 FALSE TRUE w748] -> w710
                frame 0, Default {
                  w740 = FALSE
                  # "XYZ within limits, no move"
                }
                frame 1 {
                  # "X or Y outside limit, move XY"
                }
                frame 2 {
                  # "Sigma X / Y outside limit, move Z"
                }
                frame 3 {
                  w748 = TRUE
                  # "XYZ outside limit, move all"
                }
              }
              "XY Move" <- w711
              "Z Move" <- w710
            }
            frame "Check Drift cc" {
              w758 = Stage_Actions."Get Position" ("Actions")
              n416 = Get Notifier Status(notifier=w798) -> (notifier out=w766:refnum<notifier>, current notification=w784:T8)  [unwired: 1 in, 3 out]
              n417 = call "Stages Messenger.vi"("Stage Notifier Name"=w757, "Actions"=w758) -> ("Positions"=w755:dbl[])  [unwired: 10 in, 3 out]
              n418 = call "Stages Messenger.vi"("Stage Notifier Name"=w756, "Actions"=w758) -> ("Positions"=w759:dbl[])  [unwired: 10 in, 3 out]
              n419 = Index Array(array=w755, index #1=0 ("index"), index #2=1 ("index")) -> (element #1=w750:dbl, element #2=w751:dbl)
              n420 = Index Array(array=w759, index=0) -> (element=w752:dbl)
              n421 = local write "Z Axis Position (µm)"(w752) -> ()
              n422 = local write "Y Axis Position (µm)"(w751) -> ()
              n423 = local write "X Axis Position (µm)"(w750) -> ()
              n424 = Unbundle By Name(w784) -> ("XY Correction Active"=w774:bool, "XY Drift Threshold"=w801:dbl, "PID Values"=w799:dbl[])
              n425 = local read "Measured Y Position cc (px)"() -> (w795:dbl)
              n426 = local read "Measured X Position cc (px)"() -> (w796:dbl)
              n427 = Unbundle By Name(w784) -> ("Z Correction Active"=w775:bool, "Z Drift Threshold"=w777:dbl, "PID Values"=w783:dbl[])
              n428 = local read "Target X Position cc (px)"() -> (w794:dbl)
              n429 = local read "Target Y Position cc (px)"() -> (w793:dbl)
              n430 = Array To Cluster(array=w799) -> (cluster=w800:T20)
              n431 = local read "pixel size (µm)"() -> (w802:dbl)
              n432 = Array To Cluster(array=w783) -> (cluster=w782:T20)
              n433 = Build Array(w800) -> (w797:T21)
              n434 = Build Array(w794, w793) -> (w791:dbl[])
              n435 = Build Array(w796, w795) -> (w792:dbl[])
              n436 = local read "Measured Z (µm)"() -> (w779:dbl)
              n437 = local read "Target Z (µm)"() -> (w780:dbl)
              n438 = Divide(x=w801, y=w802) -> (x/y=w789:dbl)
              n439 = Subtract(x=w792, y=w791) -> (x-y=w790:dbl[])
              n440 = call-poly <vilib>:"PID.vi"("PID gains"=w797, "process variable"=w792, "setpoint"=w791) -> ("output"=→"dxy (px)":dbl[])  [unwired: 7 in, 1 out]
              n441 = Build Array(w789, w789) -> (w788:dbl[])
              n442 = Absolute Value(x=w790) -> (abs(x)=w787:dbl[])
              n443 = Subtract(x=w779, y=w780) -> (x-y=w781:dbl)
              n444 = call-poly <vilib>:"PID.vi"("PID gains"=w782, "process variable"=w779, "setpoint"=w780) -> ("dt out (s)"=→"dt z (s)":dbl, "output"=→"dz (µm)":dbl)  [unwired: 7 in]
              n445 = Greater?(x=w787, y=w788) -> (0:w786:bool[])
              n446 = Absolute Value(x=w781) -> (abs(x)=w778:dbl)
              n447 = Or Array Elements(Boolean array=w786) -> (logical OR=w785:bool)
              n448 = Greater?(x=w778, y=w777) -> (0:w776:bool)
              n449 = And(x=w774, y=w785) -> (x .and. y?=w769:bool)
              n450 = And(x=w775, y=w776) -> (x .and. y?=w768:bool)
              n451 = Build Array(w769, w768) -> (w770:bool[])
              n452 = Boolean Array To Number(Boolean array=w770) -> (number=w771:u32)
              n453 = case shown="0, Default" w771 {
                tunnel: [4Pi_Obj_Lock_-_Actions."Update Plots" ("x") 4Pi_Obj_Lock_-_Actions."Move XY" ("x") 4Pi_Obj_Lock_-_Actions."Move Z" ("x") 4Pi_Obj_Lock_-_Actions."Move XYZ" ("x")] -> w767
                tunnel: [w803 TRUE FALSE w811] -> w765
                tunnel: [w803 FALSE TRUE w811] -> w764
                frame 0, Default {
                  w803 = FALSE
                  # "XYZ within limits, no move"
                }
                frame 1 {
                  # "X or Y outside limit, move XY"
                }
                frame 2 {
                  # "Sigma X / Y outside limit, move Z"
                }
                frame 3 {
                  w811 = TRUE
                  # "XYZ outside limit, move all"
                }
              }
              n454 = local write "XY Move"(w765) -> ()
              n455 = local write "Z Move"(w764) -> ()
            }
            frame "Check Drift cc z" {
              n456 = Get Notifier Status(notifier=w836) -> (notifier out=w824:refnum<notifier>, current notification=w835:T8)  [unwired: 1 in, 3 out]
              n457 = call "Stages Messenger.vi"("Stage Notifier Name"=w817, "Actions"=Stage_Actions."Get Position") -> ("Positions"=w819:dbl[])  [unwired: 10 in, 3 out]
              n458 = Index Array(array=w819, index=0) -> (element=w816:dbl)
              n459 = local write "Z Axis Position (µm)"(w816) -> ()
              n460 = Unbundle By Name(w835) -> ("Z Correction Active"=w826:bool, "Z Drift Threshold"=w828:dbl, "PID Values"=w834:dbl[])
              n461 = Array To Cluster(array=w834) -> (cluster=w833:T20)
              n462 = local read "Measured Z (µm)"() -> (w830:dbl)
              n463 = local read "Target Z (µm)"() -> (w831:dbl)
              n464 = Subtract(x=w830, y=w831) -> (x-y=w832:dbl)
              n465 = call-poly <vilib>:"PID.vi"("PID gains"=w833, "process variable"=w830, "setpoint"=w831) -> ("dt out (s)"=w813:dbl, "output"=w814:dbl)  [unwired: 7 in]
              n466 = Absolute Value(x=w832) -> (abs(x)=w829:dbl)
              n467 = local write "dz (µm)"(w814) -> ()
              n468 = local write "dt z (s)"(w813) -> ()
              n469 = Greater?(x=w829, y=w828) -> (0:w827:bool)
              n470 = And(x=w826, y=w827) -> (x .and. y?=w815:bool)
              n471 = case shown="True" w815 {
                tunnel: [4Pi_Obj_Lock_-_Actions."Update Plots" ("x") 4Pi_Obj_Lock_-_Actions."Move Z" ("x")] -> w825
                tunnel: [FALSE TRUE] -> w823
                frame False {
                  # "XYZ within limits, no move"
                }
                frame True {
                  # "Sigma X / Y outside limit, move Z"
                }
              }
              n472 = local write "Z Move"(w823) -> ()
            }
            frame "Check Drift cc xy" {
              n473 = Get Notifier Status(notifier=w870) -> (notifier out=w853:refnum<notifier>, current notification=w856:T8)  [unwired: 1 in, 3 out]
              n474 = call "Stages Messenger.vi"("Stage Notifier Name"=w848, "Actions"=Stage_Actions."Get Position") -> ("Positions"=w847:dbl[])  [unwired: 10 in, 3 out]
              n475 = Index Array(array=w847, index #1=0 ("index"), index #2=1 ("index")) -> (element #1=w843:dbl, element #2=w844:dbl)
              n476 = local write "Y Axis Position (µm)"(w844) -> ()
              n477 = local write "X Axis Position (µm)"(w843) -> ()
              n478 = Unbundle By Name(w856) -> ("XY Correction Active"=w855:bool, "XY Drift Threshold"=w873:dbl, "PID Values"=w871:dbl[])
              n479 = local read "Measured Y Position cc (px)"() -> (w867:dbl)
              n480 = local read "Measured X Position cc (px)"() -> (w868:dbl)
              n481 = local read "Target X Position cc (px)"() -> (w866:dbl)
              n482 = local read "Target Y Position cc (px)"() -> (w865:dbl)
              n483 = Array To Cluster(array=w871) -> (cluster=w872:T20)
              n484 = local read "pixel size (µm)"() -> (w874:dbl)
              n485 = Build Array(w872) -> (w869:T21)
              n486 = Build Array(w866, w865) -> (w863:dbl[])
              n487 = Build Array(w868, w867) -> (w864:dbl[])
              n488 = Divide(x=w873, y=w874) -> (x/y=w861:dbl)
              n489 = Subtract(x=w864, y=w863) -> (x-y=w862:dbl[])
              n490 = call-poly <vilib>:"PID.vi"("PID gains"=w869, "process variable"=w864, "setpoint"=w863) -> ("output"=w842:dbl[])  [unwired: 7 in, 1 out]
              n491 = Build Array(w861, w861) -> (w860:dbl[])
              n492 = Absolute Value(x=w862) -> (abs(x)=w859:dbl[])
              n493 = Greater?(x=w859, y=w860) -> (0:w858:bool[])
              n494 = local write "dxy (px)"(w842) -> ()
              n495 = Or Array Elements(Boolean array=w858) -> (logical OR=w857:bool)
              n496 = And(x=w855, y=w857) -> (x .and. y?=w841:bool)
              n497 = case shown="False" w841 {
                tunnel: [4Pi_Obj_Lock_-_Actions."Get Current Z Position" ("x") 4Pi_Obj_Lock_-_Actions."Move XY" ("x")] -> w854
                tunnel: [FALSE TRUE] -> w852
                frame False {
                }
                frame True {
                  # "X or Y outside limit, move XY"
                }
              }
              n498 = local write "XY Move"(w852) -> ()
            }
            frame "Move XYZ", "Move XY" {
              w905 = 2.0
              # "Initial XY stage positions"
              # "Check if move will go beyond ±2 µm of the original positions"
              n499 = case shown="False" FALSE {
                tunnel: w889 -> [_ w926]
                tunnel: [w924 w925] -> w884
                frame False {
                  n500 = local read "dxy (px)"() -> (w924:dbl[])
                }
                frame True {
                  # "Get XY Diff Values"
                  n501 = Array Subset(array=w926, index (row)=0 ("index"), length (row)=2 ("length"), index (col)=2 ("index")) -> (w927:dbl[][])  [unwired: 1 in]
                  n502 = Index Array(array=w927, index (col)=0 ("disabled index (col)")) -> (element=w925:dbl[])  [unwired: 1 in]
                }
              }
              n503 = Get Notifier Status(notifier=w922) -> (notifier out=w921:refnum<notifier>, current notification=w920:T8)  [unwired: 1 in, 3 out]
              n504 = Unbundle By Name(w920) -> ("Abort If Error"=w913:bool, "XY Stage Move Limit (µm)"=w916:dbl)
              n505 = Array Subset(array=w889, index (row)=0 ("index"), length (row)=2 ("length"), index (col)=3 ("index"), length (col)=1 ("length")) -> (w888:dbl[][])
              n506 = Index Array(array=w888, index (col)=0 ("disabled index (col)")) -> (element=w886:dbl[])  [unwired: 1 in]
              n507 = Build Array("X Update Scale Factor", "Y Update Scale Factor") -> (w880:dbl[])
              n508 = Multiply(x=w884, y=w880) -> (x*y=w883:dbl[])
              n509 = call "Stages Messenger.vi"("Stage Notifier Name"=w897, "Actions"=Stage_Actions."Get Position") -> ("Stage Notifier Name (Dup)"=w896:string, "Positions"=w895:dbl[])  [unwired: 10 in, 2 out]
              n510 = call "4Pi Obj Lock - Rotate Flip XY.vi"("XY Amounts"=w883, "Flip XY"="Flip XY Axis", "Invert X"="Invert X Axis", "Invert Y"="Invert Y Axis") -> ("45° Rotated XY"=w885:dbl[])  [unwired: 11 in]
              n511 = Add(x=w895, y=w885) -> (x+y=w894:dbl[])
              n512 = Add(x=w886, y=w905) -> (x+y=w903:dbl[])
              n513 = Subtract(x=w886, y=w905) -> (x-y=w904:dbl[])
              n514 = Absolute Value(x=w885) -> (abs(x)=w915:dbl[])
              n515 = Greater?(x=w916, y=w915) -> (0:w914:bool[])
              n516 = In Range and Coerce(upper limit=w903, x=w894, lower limit=w904) -> (In Range?=w902:bool[])  [unwired: 1 out]
              n517 = And Array Elements(Boolean array=w914) -> (logical AND=w901:bool)
              n518 = And Array Elements(Boolean array=w902) -> (logical AND=w899:bool)
              n519 = And(x=w901, y=w899) -> (x .and. y?=w900:bool)
              n520 = Not(x=w900) -> (.not. x?=→"Move Limit Error":bool)
              n521 = case shown="True" w900 {
                tunnel: w885 -> [_ w942]
                tunnel: w913 -> [w936 _]
                tunnel: [w934 4Pi_Obj_Lock_-_Actions."Get Current Z Position" ("f")] -> w912
                tunnel: w896 -> [_ w941]
                tunnel: [dbl[] [-1.0, -1.0] ("Positions") w940] -> w910
                frame False {
                  n522 = Select(t=4Pi_Obj_Lock_-_Actions."Abort" ("x"), s=w936, f=4Pi_Obj_Lock_-_Actions."Get Current Z Position") -> (s? t:f=w934:T6)
                }
                frame True {
                  n523 = call "Stages Messenger.vi"("Stage Notifier Name"=w941, "Actions"=Stage_Actions."MVR", "Setpoint"=w942, "Axis"=bool[] [TRUE, TRUE], "Exit While Busy?"=FALSE) -> ("Positions"=w940:dbl[])  [unwired: 7 in, 3 out]
                  n524 = Wait (ms)(milliseconds to wait=u32 100) -> ()  [unwired: 1 out]
                }
              }
              n525 = Index Array(array=w910, index #1=0 ("index"), index #2=1 ("index")) -> (element #1=→"X Axis Position (µm)":dbl, element #2=→"Y Axis Position (µm)":dbl)
            }
            frame "Move Z" {
              w958 = 2.0 ("y")
              # "Initial Z stage position"
              n526 = Get Notifier Status(notifier=w976) -> (notifier out=w975:refnum<notifier>, current notification=w977:T8)  [unwired: 1 in, 3 out]
              n527 = case shown="False" FALSE {
                tunnel: [w979 w982] -> w970
                tunnel: w952 -> [_ w980]
                frame False {
                  n528 = local read "dz (µm)"() -> (w979:dbl)
                }
                frame True {
                  w981 = 0 ("disabled index (col)")
                  # "Get sx/sy Diff Value"
                  n529 = Array Subset(array=w980, index (row)=2 ("index"), length (row)=1 ("length"), index (col)=2 ("index"), length (col)=1 ("length")) -> (w984:dbl[][])
                  n530 = Index Array(array=w984, index (row)=w981, index (col)=w981) -> (element=w982:dbl)
                }
              }
              n531 = Index Array(array=w952, index (row)=2, index (col)=3 ("disabled index (col)")) -> (element=w949:dbl)
              n532 = Unbundle By Name(w977) -> ("Abort If Error"=w957:bool, "Z Stage Move Limit (µm)"=w962:dbl)
              n533 = Multiply(x=w970, y="Z Update Scale Factor") -> (x*y=w967:dbl)
              n534 = Add(x=w949, y=w958) -> (x+y=w964:dbl)
              n535 = Subtract(x=w949, y=w958) -> (x-y=w963:dbl)
              n536 = call "Stages Messenger.vi"("Stage Notifier Name"=w973, "Actions"=Stage_Actions."Get Position") -> ("Stage Notifier Name (Dup)"=w959:string, "Positions"=w971:dbl[])  [unwired: 10 in, 2 out]
              n537 = Negate(x=w967) -> (-x=w968:dbl)
              n538 = Select(t=w968, s="Invert Z Axis", f=w967) -> (s? t:f=w948:dbl)
              n539 = Index Array(array=w971, index=0) -> (element=w969:dbl)
              n540 = Absolute Value(x=w948) -> (abs(x)=w947:dbl)
              n541 = Add(x=w948, y=w969) -> (x+y=w965:dbl)
              n542 = Greater?(x=w962, y=w947) -> (0:w961:bool)
              n543 = In Range and Coerce(upper limit=w964, x=w965, lower limit=w963) -> (In Range?=w960:bool)  [unwired: 1 out]
              n544 = And(x=w961, y=w960) -> (x .and. y?=w956:bool)
              n545 = Not(x=w956) -> (.not. x?=w955:bool)
              n546 = case shown="True" w956 {
                tunnel: w959 -> [_ w1002]
                tunnel: w957 -> [w991 _]
                tunnel: w948 -> [_ w1001]
                tunnel: [w990 4Pi_Obj_Lock_-_Actions."Update Plots" ("x")] -> w954
                tunnel: [-1.0 ("Position") w996] -> w953
                frame False {
                  n547 = Select(t=4Pi_Obj_Lock_-_Actions."Abort" ("x"), s=w991, f=4Pi_Obj_Lock_-_Actions."Update Plots") -> (s? t:f=w990:T6)
                }
                frame True {
                  n548 = Build Array(w1001) -> (w1000:dbl[])
                  n549 = call "Stages Messenger.vi"("Stage Notifier Name"=w1002, "Actions"=Stage_Actions."MVR", "Setpoint"=w1000, "Axis"=bool[] [TRUE], "Exit While Busy?"=FALSE) -> ("Positions"=w998:dbl[])  [unwired: 7 in, 3 out]
                  n550 = Wait (ms)(milliseconds to wait=u32 100) -> ()  [unwired: 1 out]
                  n551 = Index Array(array=w998, index=0) -> (element=w996:dbl)
                }
              }
              "Z Axis Position (µm)" <- w953
              n552 = local write "Move Limit Error"(w955) -> ()
            }
            frame "Update Plots" {
              (unwired) 0 ("index")
              # "Current Values"
              # "Target Values"
              n553 = Get Notifier Status(notifier=w1087) -> (notifier out=w1086:refnum<notifier>, current notification=w1088:T8)  [unwired: 1 in, 3 out]
              n554 = Unbundle By Name(w1088) -> ("Z Drift Threshold"=w1079:dbl, "XY Drift Threshold"=w1078:dbl)
              n555 = local read "X Axis Position (µm)"() -> (w1073:dbl)
              n556 = local read "Y Axis Position (µm)"() -> (w1072:dbl)
              n557 = local read "Z Axis Position (µm)"() -> (w1071:dbl)
              n558 = Index Array(array=w1068, index (col)=0 ("disabled index (col)")) -> (element=w1065:dbl[])  [unwired: 1 in]
              n559 = Index Array(array=w1068, index (col)=1 ("disabled index (col)")) -> (element=w1066:dbl[])  [unwired: 1 in]
              n560 = Index Array(array=w1068, index (col)=3 ("disabled index (col)")) -> (element=w1069:dbl[])  [unwired: 1 in]
              n561 = Subtract(x=w1066, y=w1065) -> (x-y=w1064:dbl[])
              n562 = local read "Measured Y Position cc (px)"() -> (w1051:dbl)
              n563 = local read "Measured X Position cc (px)"() -> (w1050:dbl)
              n564 = local read "Target X Position cc (px)"() -> (w1052:dbl)
              n565 = local read "Target Y Position cc (px)"() -> (w1053:dbl)
              n566 = Build Array(w1073, w1072, w1071) -> (w1070:dbl[])
              n567 = Index Array(array=w1064, index #1=0 ("index"), index #2=1 ("index"), index #3=2 ("index")) -> (element #1=w1049:dbl, element #2=w1048:dbl, element #3=w1006:dbl)
              n568 = Subtract(x=w1070, y=w1069) -> (x-y=w1067:dbl[])
              n569 = Build Array(w1049, w1048) -> (w1038:dbl[])
              n570 = Index Array(array=w1067, index #1=0 ("index"), index #2=1 ("index"), index #3=2 ("index")) -> (element #1=w1031:dbl, element #2=w1030:dbl, element #3=w1056:dbl)
              n571 = Build Array(w1050, w1051) -> (w1054:dbl[])
              n572 = Build Array(w1052, w1053) -> (w1055:dbl[])
              n573 = Build Array(w1031, w1030) -> (w1024:dbl[])
              n574 = Subtract(x=w1054, y=w1055) -> (x-y=w1047:dbl[])
              n575 = Square Root(x=2.0) -> (sqrt(x)=w1026:dbl)
              n576 = Select(t=w1038, s=FALSE, f=w1047) -> (s? t:f=w1045:dbl[])
              n577 = Divide(x=w1024, y=w1026) -> (x/y=w1025:dbl[])
              n578 = Multiply(x="pixel size (µm)", y=w1038) -> (x*y=w1034:dbl[])
              n579 = Multiply(x="pixel size (µm)", y=w1045) -> (x*y=w1044:dbl[])
              n580 = Index Array(array=w1025, index #1=0 ("index"), index #2=1 ("index")) -> (element #1=w1023:dbl, element #2=w1022:dbl)
              n581 = Index Array(array=w1044, index #1=0 ("index"), index #2=1 ("index")) -> (element #1=w1041:dbl, element #2=w1040:dbl)
              n582 = Index Array(array=w1034, index #1=0 ("index"), index #2=1 ("index")) -> (element #1=w1033:dbl, element #2=w1032:dbl)
              n583 = local read "Invert X Axis"() -> (w1012:bool)
              n584 = Add(x=w1023, y=w1022) -> (x+y=w1021:dbl)
              n585 = Subtract(x=w1023, y=w1022) -> (x-y=w1015:dbl)
              n586 = Negate(x=w1021) -> (-x=w1016:dbl)
              n587 = local read "Invert Y Axis"() -> (w1011:bool)
              n588 = Negate(x=w1015) -> (-x=w1019:dbl)
              n589 = Negate(x=w1016) -> (-x=w1020:dbl)
              n590 = local read "Flip XY Axis"() -> (w1013:bool)
              n591 = Select(t=w1019, s=w1011, f=w1015) -> (s? t:f=w1017:dbl)
              n592 = Select(t=w1020, s=w1012, f=w1016) -> (s? t:f=w1018:dbl)
              n593 = Build Array(w1018, w1017) -> (w1014:dbl[])
              n594 = case shown="True" w1013 {
                tunnel: w1014 -> [w1091 w1093]
                tunnel: [w1091 w1092] -> w1009
                frame False {
                }
                frame True {
                  n595 = Reverse 1D Array(array=w1093) -> (reversed array=w1092:dbl[])
                }
              }
              n596 = Index Array(array=w1009, index #2=1 ("index")) -> (element #1=w1008:dbl, element #2=w1007:dbl)  [unwired: 1 in]
              n597 = call "4Pi Obj Lock - 1 Values Organize Plot Data.vi"("Target 01"=0.0, "Value Limit"=w1078, "Current 2"=w1033, "Current 01"=w1041, "Stage Pos"=w1008) -> ("plot value"=→"X Target and Fit Position (µm)":T2)  [unwired: 10 in]
              n598 = Multiply(x=w1006, y=0.4) -> (x*y=w1004:dbl)
              n599 = local read "Measured Z (µm)"() -> (w1059:dbl)
              n600 = call "4Pi Obj Lock - 1 Values Organize Plot Data.vi"("Target 01"=0.0, "Value Limit"=w1078, "Current 2"=w1032, "Current 01"=w1040, "Stage Pos"=w1007) -> ("plot value"=→"Y Target and Fit Position (µm)":T2)  [unwired: 10 in]
              n601 = Select(t=w1004, s=FALSE, f=w1059) -> (s? t:f=w1057:dbl)
              n602 = call "4Pi Obj Lock - 1 Values Organize Plot Data.vi"("Target 01"=0.0, "Value Limit"=w1079, "Current 2"=w1004, "Current 01"=w1057, "Stage Pos"=w1056) -> ("plot value"=→"Z Target and Fit Value (µm)":T2)  [unwired: 10 in]
            }
            frame "Delay" {
              n603 = Get Notifier Status(notifier=w1099) -> (notifier out=w1097:refnum<notifier>, current notification=w1100:T8)  [unwired: 1 in, 3 out]
              n604 = Unbundle By Name(w1100) -> ("Update Delay (ms)"=w1096:i32)
              n605 = while {
                tunnel: w1097 -> [w1112]
                tunnel: w1096 -> [w1109]
                tunnel: [w1105] -> w1095
                i -> [w1110]
                stop <- w1103 stop-if-true
                n606 = Get Notifier Status(notifier=w1112) -> (notifier out=w1105:refnum<notifier>, current notification=w1108:T8)  [unwired: 1 in, 3 out]
                n607 = Greater Or Equal?(x=w1110, y=w1109) -> (x >= y?=w1104:bool)
                n608 = Wait (ms)(milliseconds to wait=u32 1) -> ()  [unwired: 1 out]
                n609 = Unbundle By Name(w1108) -> ("Actions"=w1107:T6)
                n610 = Equal?(x=w1107, y=4Pi_Obj_Lock_-_Actions."Abort") -> (x = y?=w1102:bool)
                n611 = Or(x=w1102, y=w1104) -> (x .or. y?=w1103:bool)
              }
            }
            frame "Abort" {
              w1116 = 0.0 ("Target X Position (px)")
              n612 = Get Notifier Status(notifier=w1122) -> (notifier out=w1126:refnum<notifier>, current notification=w1125:T8)  [unwired: 1 in, 3 out]
              n613 = call "Camera Messenger.vi"("Notifier Name"=w1114, "General Camera Actions"=Generic_Camera_Actions."Abort") -> ()  [unwired: 8 in, 6 out]
              n614 = Bundle By Name(cluster=w1125, "Running?"=FALSE, "Actions"=4Pi_Obj_Lock_-_Actions."Exit Loop") -> (w1123:T8)
              n615 = Send Notification(notification=w1123, notifier=w1126) -> (notifier out=w1121:refnum<notifier>)  [unwired: 1 in, 1 out]
              n616 = local write "Start Lock"(FALSE ("Start Lock")) -> ()
              n617 = local write "Measured X Position (px)"(w1116) -> ()
              n618 = local write "Measured Y Position (px)"(w1116) -> ()
              n619 = local write "Target X Position (px)"(w1116) -> ()
              n620 = local write "Target Y Position (px)"(w1116) -> ()
              n621 = local write "Measured sx/sy"(w1116) -> ()
              n622 = local write "Target sx/sy"(w1116) -> ()
            }
            frame "Exit Loop" {
            }
            frame "Quit" {
              n623 = Get Notifier Status(notifier=w1132) -> (notifier out=w1131:refnum<notifier>, current notification=w1139:T8)  [unwired: 1 in, 3 out]
              n624 = Unbundle By Name(w1139) -> ("Ref Stack (SGL)"=w1138:T9[], "Cur Image (SGL)"=w1137:T9, "Tmp Image FFT (CSG)"=w1136:T9[], "CC Image (SGL)"=w1135:T9, "Ref FFT Stack (CSG)"=w1133:T9[])
              n625 = Release Notifier(notifier=w1131, force destroy? (F)=TRUE) -> ()  [unwired: 1 in, 3 out]
              n626 = Build Array (concatenate)(w1138, w1137, w1136, w1135, w1133) -> (w1134:T9[])
              n627 = for {
                tunnel: w1134 -> [w1144] mode=indexing
                n628 = call "IMAQ Dispose"("Image"=w1144) -> ()  [unwired: 5 in, 1 out]
              }
            }
          }
          n629 = Get Notifier Status(notifier=w234) -> (current notification=w233:T8, error out=w228:errorcluster)  [unwired: 1 in, 3 out]
          n630 = Unbundle By Name(w233) -> ("Actions"=w232:T6)
          n631 = Unbundle By Name(w228) -> ("status"=w226:bool)
          n632 = Equal?(x=w231, y=w232) -> (x = y?=w227:bool)
          n633 = Or(x=w227, y=w226) -> (x .or. y?=w225:bool)
          n634 = Select(t=w231, s=w225, f=w230) -> (s? t:f=w229:T6)
        }
      }
      n635 = local write "Quit"(w208) -> ()
    }
    frame Error {
    }
  }
  n636 = control-ref of="This VI"() -> (w87:refnum<vi>)
  n637 = property class="VI"(reference=w87) -> (reference out=w96:refnum<vi>, "Panel"=w88:refnum<vi>)  [unwired: 1 in, 1 out]
  n638 = property class="Pnl"(reference=w88) -> ("Decos[]"=w86:refnum<vi>[], "Panes[]"=w92:refnum<vi>[])  [unwired: 1 in, 2 out]
  n639 = Array Size(array=w86) -> (size(s)=w84:i32)
  n640 = Decrement(x=w84) -> (x-1=w85:i32)
  n641 = Index Array(array=w92, index=0) -> (element=w91:refnum<vi>)
  n642 = Index Array(array=w86, index=w85) -> (element=w94:refnum<vi>)
  n643 = property class="VI"(reference=w96) -> (reference out=w98:refnum<vi>, "Front Panel.PanelBounds"=w99:T22)  [unwired: 1 in, 1 out]
  n644 = property class="Decor"(reference=w94) -> ("Bounds"=w97:T23)  [unwired: 1 in, 2 out]
  n645 = property class="Pane"(reference=w91, "Origin"=T11 {"Horizontal"=0, "Vertical"=0}, "HorizScrollbarVisibility"=w95, "VertScrollbarVisibility"=w95) -> ()  [unwired: 1 in, 2 out]
  n646 = Unbundle By Name(w97) -> ("Width"=w102:u32, "Height"=w105:u32)
  n647 = control-ref of="Quit"() -> (w89:refnum<vi>)
  n648 = To Word Integer(number=w102) -> (16bit integer=w104:i16)
  n649 = To Word Integer(number=w105) -> ()  [unwired: 1 out]
  n650 = property class="Bool (strict)"(reference=w89) -> ("Height"=w107:u32, "Top"=w108:i32)  [unwired: 1 in, 2 out]
  n651 = Unbundle By Name(w99) -> ("Left"=w101:i16, "Top"=w112:i16)
  n652 = To Word Integer(number=w107) -> (16bit integer=w110:i16)
  n653 = To Word Integer(number=w108) -> (16bit integer=w111:i16)
  n654 = Add(x=w101, y=w104) -> (x+y=w103:i16)
  n655 = Compound Arithmetic op=ADD(w112, w110, w111, i16 12 ("y")) -> (w106:i16)
  n656 = Bundle By Name(cluster=w99, "Right"=w103, "Bottom"=w106) -> (w100:T22)
  n657 = property class="VI"(reference=w98, "Front Panel.PanelBounds"=w100) -> ()  [unwired: 1 in, 2 out]
